vi "温度控制 - WK12.vi"(7 "CSM Name":string="WK1") -> ()   [LabVIEW 2017, in "UI-温度控制.lvlib"]
doc: "本范例执行串口读写操作。串口设置的参数必须匹配连接仪器或设备的参数。“VISA配置串口”VI可设置配置参数。前面板显示的控件可用于配置基本参数，如波特率、数据位和校验。VI会将VISA资源名称传递至其他VI以便执行相关操作。“VISA写入”函数将发送一个命令至串行设备，“VISA读取”函数将返回基于该命令的数据。“VISA关闭”函数可关闭该串行设备的引用。关闭引用十分重要，否则可能导致无法通过该端口进行进一步通信。"
uses:
  <userlib>/_NEVSTOP/Communicable State Machine(CSM)/Communicable State Machine.lvlib
  <userlib>/_NEVSTOP/Communicable State Machine(CSM)/addons/MassData-Parameter/CSM MassData Parameter Support.lvlib
  <userlib>/_NEVSTOP/Communicable State Machine(CSM)/addons/INI-Static-Variable-Support/INI-Static-Variable-Support.lvlib
  <userlib>/_NEVSTOP/Communicable State Machine(CSM)/addons/Watchdog/CSM Watchdog.lvlib
  <userlib>/_NEVSTOP/Communicable State Machine(CSM)/addons/Logger/CSM File Logger.lvlib
  e87f5527-76ec-45cd-8a15-2e3ba2958834.vi
  e40b3fcb-6c9f-41ae-97ff-bcb9991e0652.vi
  620e82e9-b677-4d25-b56c-4b090e123e3d.vi
  fecb341a-c865-4baa-9917-6b90415d6ef9.vi
  afd7753c-ea30-4e5b-9716-29bc73ab5d02.vi
  9a199716-2ffa-4f43-b9de-bb583d0dc84c.vi
  b5fe0464-1048-4df8-950b-6816aac68042.vi
  <userlib>/_NEVSTOP/Communicable State Machine(CSM)/_Polymophic/CSM - Replace Marks in Messages.vi
  7f493404-46e2-4a42-937c-85a599ffd008.vi
  3c0606d2-39f9-4349-a74d-1248628ec5a5.vi
  b1075206-a0bc-4c2c-8117-03daddfb89bc.vi
  12798cb0-d503-413b-8ceb-4a5576430bcb.vi
  22b4bb12-f94e-4276-9d0b-49463fdbebaf.vi
  87263e8e-d87a-4015-b0d9-f89f6746087b.vi
  45ac6a38-59b2-4408-864e-de2893445c95.vi
  3f8d9458-3e99-4457-8efa-55d1ef2330f2.vi
  bd3177e1-6bd6-42ad-a258-ed35146a2f34.vi
  acea6df9-f425-4d5c-b033-3243991d638c.vi
  611bdd8b-2aca-4a53-81a9-536b5b4081e0.vi
  6c66f1b3-0c4e-481a-bccf-761e4204c7a2.vi
  bd3fa8c0-2a07-4348-928a-5492c50b8d1d.vi
  bfd69444-e477-482d-b4ce-b6780147d2f5.vi
  3eee923a-0692-424c-8c25-dbf31775acba.vi
  026bd4a5-6a46-4a68-819b-9f168641a175.vi
  6fdd3ccc-b7af-4740-b642-363912b39baa.vi
  3bdb7142-561a-47bb-abd8-0318bec92597.vi
  dc7ef564-96da-43a3-866d-645d9c897f58.vi
  <vilib>/Instr/_visa.llb/VISA Configure Serial Port (Instr).vi
  6094d1ba-01c9-4f0f-81c2-2bfc5faa83cd.vi
  36fd150c-2ad9-4592-a276-8ca334c7aa56.vi
  f347ec19-a9ab-456c-bf02-8d1d7c992b68.vi
  6f01d93e-47d7-4c16-bfcb-79e48a01ebec.vi
  9b669b8c-733c-4058-8ee2-0fdaa3bce225.vi
  b7989555-3743-433e-92bc-1f24cc67f5f4.vi
  e0d25892-2f3c-4bdd-91b3-ce78b04bde2a.vi
  7ceba0d5-fd35-45f6-9e4f-db13be910fa9.vi
  e709ab76-91cd-483a-bfeb-5221a7f7e432.vi
  <userlib>/_NEVSTOP/Communicable State Machine(CSM)/addons/INI-Static-Variable-Support/_Support/instances/_CSM - Read File Logger Configuration - v1.0.vi
  <userlib>/_NEVSTOP/Communicable State Machine(CSM)/_Polymophic/CSM - Filter Duplicated Lines.vi
  <userlib>/_NEVSTOP/Communicable State Machine(CSM)/_Polymophic/Add State(s) to Queue By BOOL(Element).vi
  52a88361-96b9-4f42-83b5-2b3a91f6fe46.vi
  6e92e572-67e2-4f23-93e9-3f2621f8ebb2.vi
  fcc43e12-244c-4800-bcec-4b40395c6c4b.vi
  b77c82fb-bb1b-4fca-94e8-a2470f067fd9.vi
  cab45986-ae3d-44a0-b15a-916822da0a04.vi
  b63380f4-522f-43f9-8c86-ff87e18121f1.vi
  e181f527-371e-42fd-b1ab-20e25477ecf6.vi
  2a5f06fa-bc14-4be7-8a56-d3603e987429.vi
  Data ColndSave/Supports/Time and Data.ctl
  Data ColndSave/Data Collection and Save.lvlib
  Supports/Device Info.ctl
  a4ed0b2b-8fbd-453e-8bc8-e71f1ca0e4fa.vi
  967289fb-03de-4dd6-8fec-445893c11e8c.vi
panel:
  in  "停止":bool
  in  "温度显示":T1(tab)
  in  "温控开关 总":bool
  in  "跟随通道 1":T2
  in  "跟随通道 2":T2
  in  "通道":bool
  in  "温控温度 B":dbl=25.0 min=-10.0 max=50.0 step=0.1 format="%.2g"
  in  "温控温度 A":dbl=25.0 min=-10.0 max=50.0 step=0.1 format="%.2g"
  in  "温度":bool
  in  "跟随偏移 2":dbl min=-10.0 max=50.0 step=0.01 format="%#.2g"
  in  "是否跟随 2":bool
  in  "跟随偏移 1":dbl min=-10.0 max=50.0 step=0.01 format="%#.2g"
  in  "是否跟随 1":bool
  in  "打开串口":bool
  in  "温控串口":refnum<visa-resource-name>="COM18"
  out "TC2":waveform(dbl)[](graph)
  out "TC1":waveform(dbl)[](graph)
  in  "温控开关 2":bool
  in  "温控开关 1":bool
  in  "温控温度 2":dbl=25.0 min=-10.0 max=50.0 step=0.1 format="%.2g"
  out "实际温度 2":dbl=25.0 format="%.2g"
  out "实际温度 1":dbl=25.0 format="%.2g"
  in  "温控温度 1":dbl=25.0 min=-10.0 max=50.0 step=0.1 format="%.2g"
  in  "Fast Mode":bool
  in  "采集间隔":dbl=0.5 min=0.05 max=50.0 step=0.1 format="%.2g"
  out "Power 2":waveform(dbl)[](graph)
  out "Power 1":waveform(dbl)[](graph)
  out "输出状态 1":T3
  out "输出状态 2":T3
  in  "电源切换 2":bool
  in  "电源切换 1":bool
  in  "输出设置 2":T4={"输出模式"=enum."加热模式", "最大输出电压"=5.0} {"最大输出电压" min=0.0001 max=10.0}
  in  "输出设置 1":T4={"输出模式"=enum."加热模式", "最大输出电压"=5.0} {"最大输出电压" min=0.0001 max=10.0}
  in  "PID 1":T5={"PID类型"=enum."PID", "P"=0.05, "I"=20.0, "D"=2.0, "PID控制间隔"=100.0, "PID计算方法"=enum."最大正向输出"}
  in  "PID 2":T5={"PID类型"=enum."PID", "P"=0.05, "I"=20.0, "D"=2.0, "PID控制间隔"=100.0, "PID计算方法"=enum."最大正向输出"}
  in  "过压/过流 2":cluster{"过压保护阈值":dbl, "过流保护阈值":dbl}={"过压保护阈值"=6.0, "过流保护阈值"=3.0}
  in  "过压/过流 1":cluster{"过压保护阈值":dbl, "过流保护阈值":dbl}={"过压保护阈值"=6.0, "过流保护阈值"=3.0}
  in  "过温 2":T6={"过温保护开关"=TRUE, "过温保护低阈值"=5.0, "过温保护高阈值"=45.0, "最低设定温度"=5.0, "最高设定温度"=45.0, "温度限速"=45.0} {"温度限速" min=0.01}
  out "保护结果 2":T7={"过压保护结果"=enum."正常", "过流保护结果"=enum."正常", "过温保护结果"=enum."正常"}
  out "保护结果 1":T7={"过压保护结果"=enum."正常", "过流保护结果"=enum."正常", "过温保护结果"=enum."正常"}
  in  "过温 1":T6={"过温保护开关"=TRUE, "过温保护低阈值"=5.0, "过温保护高阈值"=45.0, "最低设定温度"=5.0, "最高设定温度"=45.0, "温度限速"=45.0} {"温度限速" min=1e-06; "最低设定温度" min=0.0001}
  in  "温控循环功能开启":bool
  in  "子程序？":bool
  out "温控-错误输出":errorcluster
  out "温控器设备型号":string
  out "State History":string
  # "温度快切"
  # "V"
  # "A"
  # "V"
  # "A"
  # "V"
  # "V"
  # "ms"
  # "ms"
  # "℃/s"
  # "℃/s"
  # "恢复，继续运行；\n如继续报错，请检查参数，可尝试关闭串口重新打开。"
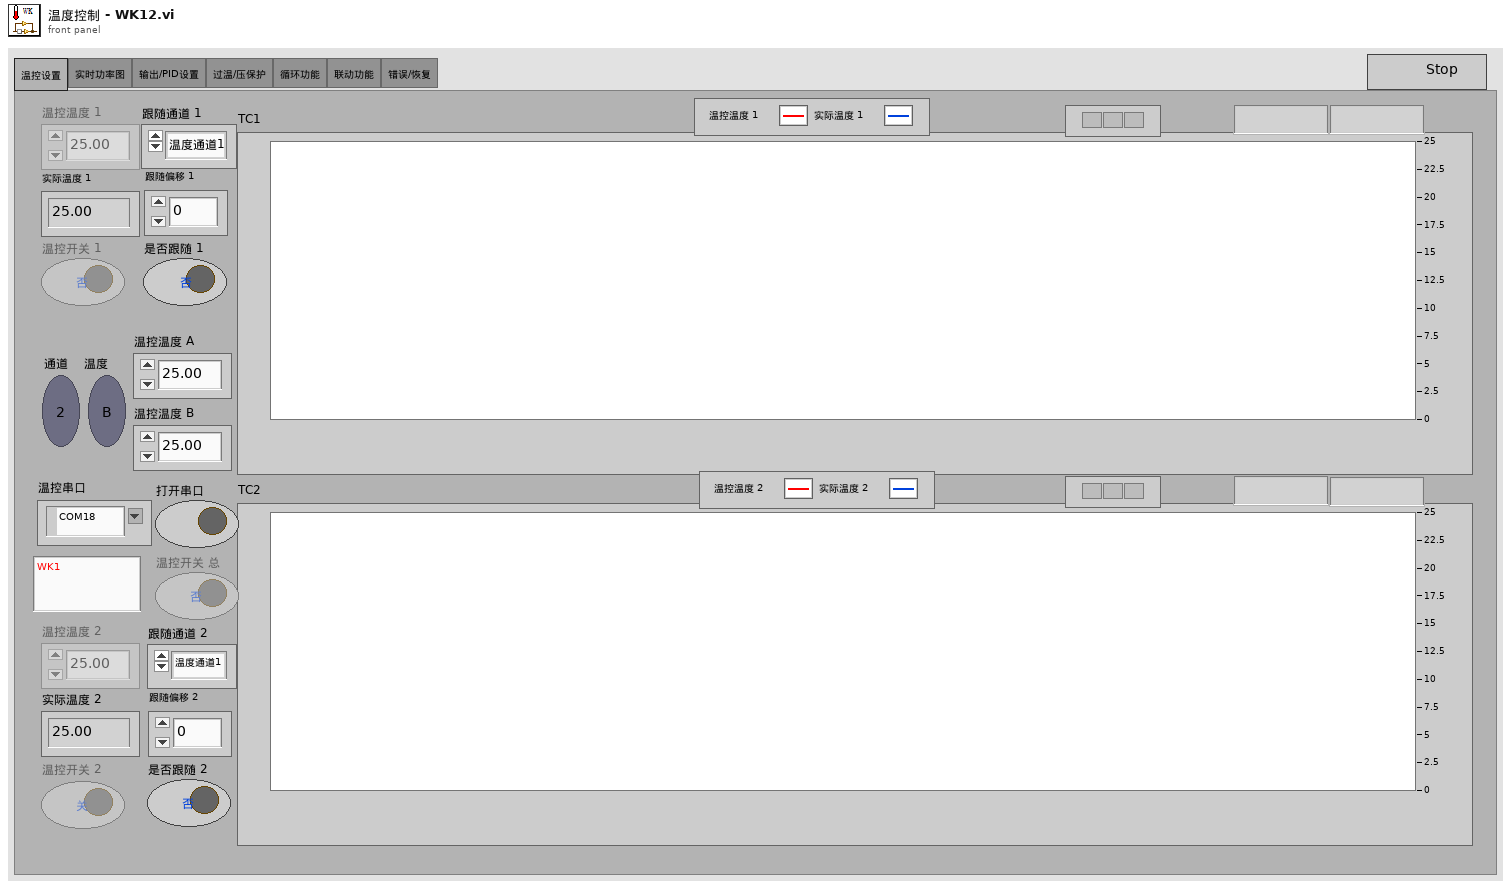
[diagram p1: front panel]
types:
  T1 = enum32{"温控设置", "实时功率图", "输出/PID设置", "过温/压保护", "循环功能", "联动功能", "错误/恢复"}
  T2 = typedef "UI-压力.lvlib/温度各项索引.ctl" = enum16{"温度通道1", "温度通道2", "温度通道3", "温度通道4", "温度通道5", "温度通道6", "温度通道7", "温度通道8", "TC1控制温度", "TC1实际温度", "TC1实际输出电压", "TC1实际输出电流", "TC1实际输出功率", "TC2控制温度", "TC2实际温度", "TC2实际输出电压", "TC2实际输出电流", "TC2实际输出功率", "压力(电压值)", "压力(g)", "步进电机位置", "温度", "湿度", "LD设定温度(度)", "LD实际温度(度)", "LD设定温度(脉冲值)", "LD实际温度(脉冲值)", "LD PWM(功率)"}
  T3 = cluster{"功率输出":enum16{"已关闭", "已打开"}, "实际输出电压":dbl, "实际输出电流":dbl}
  T4 = cluster{"输出模式":enum16{"致冷模式", "加热模式", "双向模式"}, "最大输出电压":dbl}
  T5 = cluster{"PID类型":enum16{"P", "PI", "PID"}, "P":dbl, "I":dbl, "D":dbl, "PID控制间隔":dbl, "PID计算方法":enum16{"位置式", "增量式", "最大正向输出", "最大负向输出"}}
  T6 = cluster{"过温保护开关":bool, "过温保护低阈值":dbl, "过温保护高阈值":dbl, "最低设定温度":dbl, "最高设定温度":dbl, "温度限速":dbl}
  T7 = cluster{"过压保护结果":enum16{"发现错误", "正常", "功能关闭"}, "过流保护结果":enum16{"发现错误", "正常", "功能关闭"}, "过温保护结果":enum16{"发现错误", "正常", "功能关闭"}}
  T8 = cluster{"Enable":bool, "Limit":cluster{"FileSize":i64, "FileNum":i32}, "Timestamp.Format":string, "AutoExit":bool}
  T9 = enum32{"Invalid", "Standard", "Closed", "Hidden", "Minimized", "Maximized"}
  T10 = enum32{"invalid app kind", "Development System", "Run Time System", "Student Edition", "Embedded LabVIEW", "Evaluation", "Custom"}
  T11 = typedef "Device Info.ctl" = cluster{"基本信息":cluster{"USB Port":refnum<visa-resource-name>, "采集间隔(s)":dbl}, "设备信息":cluster{"设备型号":string, "双通道设备？":bool}, "开关":cluster{"开关 1":bool, "开关 2":bool, "Fast Mode":bool}, "Control Temp":cluster{"Control Temp 1":dbl, "Control Temp 2":dbl}}
  T12 = cluster{"波特率":u32, "数据位":u16, "校验":enum16{"None", "Odd", "Even", "Mark", "Space"}, "停止位":u16, "流控制":u16}
  T13 = typedef "Communicable State Machine.lvlib/_CSM_Response Source Message.ctl" = cluster{"‘State":string, "’Arguments":string, "’Error":errorcluster}
  T14 = cluster{"Current VI Reference":refnum<vi>, "Close Panel on Exit?":bool}
  T15 = typedef "Data Collection and Save.lvlib/Time and Data.ctl" = cluster{"采集时间":timestamp, "Data":dbl[]}
  T16 = cluster{"Core":cluster{"Current VI Reference":refnum<vi>, "Close Panel on Exit?":bool}, "基本信息":cluster{"USB Port":refnum<visa-resource-name>, "采集间隔(s)":dbl}, "温控情况":cluster{"温控温度 1":dbl, "实际温度 1":dbl, "温控温度 2":dbl, "实际温度 2":dbl, "打开串口":bool}, "开关信息":cluster{"开关 1":bool, "开关 2":bool, "温控是否打开":bool}, "输出参数":cluster{"输出设置 1":cluster{"输出模式":enum16{"致冷模式", "加热模式", "双向模式"}, "最大输出电压":dbl}, "输出设置 2":cluster{"输出模式":enum16{"致冷模式", "加热模式", "双向模式"}, "最大输出电压":dbl}, "输出状态 1":cluster{"功率输出":enum16{"已关闭", "已打开"}, "实际输出电压":dbl, "实际输出电流":dbl, "实际输出功率":dbl}, "输出状态 2":cluster{"功率输出":enum16{"已关闭", "已打开"}, "实际输出电压":dbl, "实际输出电流":dbl, "实际输出功率":dbl}, "PID 1":cluster{"PID类型":enum16{"P", "PI", "PID"}, "P":dbl, "I":dbl, "D":dbl, "PID控制间隔":dbl, "PID计算方法":enum16{"位置式", "增量式", "最大正向输出", "最大负向输出"}}, "PID 2":cluster{"PID类型":enum16{"P", "PI", "PID"}, "P":dbl, "I":dbl, "D":dbl, "PID控制间隔":dbl, "PID计算方法":enum16{"位置式", "增量式", "最大正向输出", "最大负向输出"}}}, "保护":cluster{"过压/过流 1":cluster{"过压保护阈值":dbl, "过流保护阈值":dbl}, "过压/过流 2":cluster{"过压保护阈值":dbl, "过流保护阈值":dbl}, "保护结果 1":cluster{"过压保护结果":enum16{"发现错误", "正常", "功能关闭"}, "过流保护结果":enum16{"发现错误", "正常", "功能关闭"}, "过温保护结果":enum16{"发现错误", "正常", "功能关闭"}}, "保护结果 2":cluster{"过压保护结果":enum16{"发现错误", "正常", "功能关闭"}, "过流保护结果":enum16{"发现错误", "正常", "功能关闭"}, "过温保护结果":enum16{"发现错误", "正常", "功能关闭"}}, "过温 1":cluster{"过温保护开关":bool, "过温保护低阈值":dbl, "过温保护高阈值":dbl, "最低设定温度":dbl, "最高设定温度":dbl, "温度限速":dbl}, "过温 2":cluster{"过温保护开关":bool, "过温保护低阈值":dbl, "过温保护高阈值":dbl, "最低设定温度":dbl, "最高设定温度":dbl, "温度限速":dbl}}, "设备信息":cluster{"设备型号":string, "双通道设备？":bool}, "Time and Data":T15, "子程序":cluster{"子程序？":bool}}
  T17 = cluster{"过压/过流 1":cluster{"过压保护阈值":dbl, "过流保护阈值":dbl}, "过压/过流 2":cluster{"过压保护阈值":dbl, "过流保护阈值":dbl}, "保护结果 1":cluster{"过压保护结果":enum16{"发现错误", "正常", "功能关闭"}, "过流保护结果":enum16{"发现错误", "正常", "功能关闭"}, "过温保护结果":enum16{"发现错误", "正常", "功能关闭"}}, "保护结果 2":cluster{"过压保护结果":enum16{"发现错误", "正常", "功能关闭"}, "过流保护结果":enum16{"发现错误", "正常", "功能关闭"}, "过温保护结果":enum16{"发现错误", "正常", "功能关闭"}}, "过温 1":cluster{"过温保护开关":bool, "过温保护低阈值":dbl, "过温保护高阈值":dbl, "最低设定温度":dbl, "最高设定温度":dbl, "温度限速":dbl}, "过温 2":cluster{"过温保护开关":bool, "过温保护低阈值":dbl, "过温保护高阈值":dbl, "最低设定温度":dbl, "最高设定温度":dbl, "温度限速":dbl}}
  T18 = cluster{"输出设置 1":cluster{"输出模式":enum16{"致冷模式", "加热模式", "双向模式"}, "最大输出电压":dbl}, "输出设置 2":cluster{"输出模式":enum16{"致冷模式", "加热模式", "双向模式"}, "最大输出电压":dbl}, "输出状态 1":cluster{"功率输出":enum16{"已关闭", "已打开"}, "实际输出电压":dbl, "实际输出电流":dbl, "实际输出功率":dbl}, "输出状态 2":cluster{"功率输出":enum16{"已关闭", "已打开"}, "实际输出电压":dbl, "实际输出电流":dbl, "实际输出功率":dbl}, "PID 1":cluster{"PID类型":enum16{"P", "PI", "PID"}, "P":dbl, "I":dbl, "D":dbl, "PID控制间隔":dbl, "PID计算方法":enum16{"位置式", "增量式", "最大正向输出", "最大负向输出"}}, "PID 2":cluster{"PID类型":enum16{"P", "PI", "PID"}, "P":dbl, "I":dbl, "D":dbl, "PID控制间隔":dbl, "PID计算方法":enum16{"位置式", "增量式", "最大正向输出", "最大负向输出"}}}
  T19 = cluster{"温控温度 1":dbl, "实际温度 1":dbl, "温控温度 2":dbl, "实际温度 2":dbl, "打开串口":bool}
  T20 = cluster{"USB Port":refnum<visa-resource-name>, "采集间隔(s)":dbl}
  T21 = enum8{"Enabled", "Disabled", "Disabled and Grayed Out"}
  T22 = cluster{"控制温度":dbl, "时长(s)":dbl, "进度":dbl, "温控开关":bool}[]
  T23 = cluster{"PID类型":bool, "P":bool, "I":bool, "D":bool, "PID控制间隔":bool, "PID计算方法":bool}
  T24 = cluster{"过温保护开关":bool, "过温保护低阈值":bool, "过温保护高阈值":bool, "最低设定温度":bool, "最高设定温度":bool, "温度限速":bool}
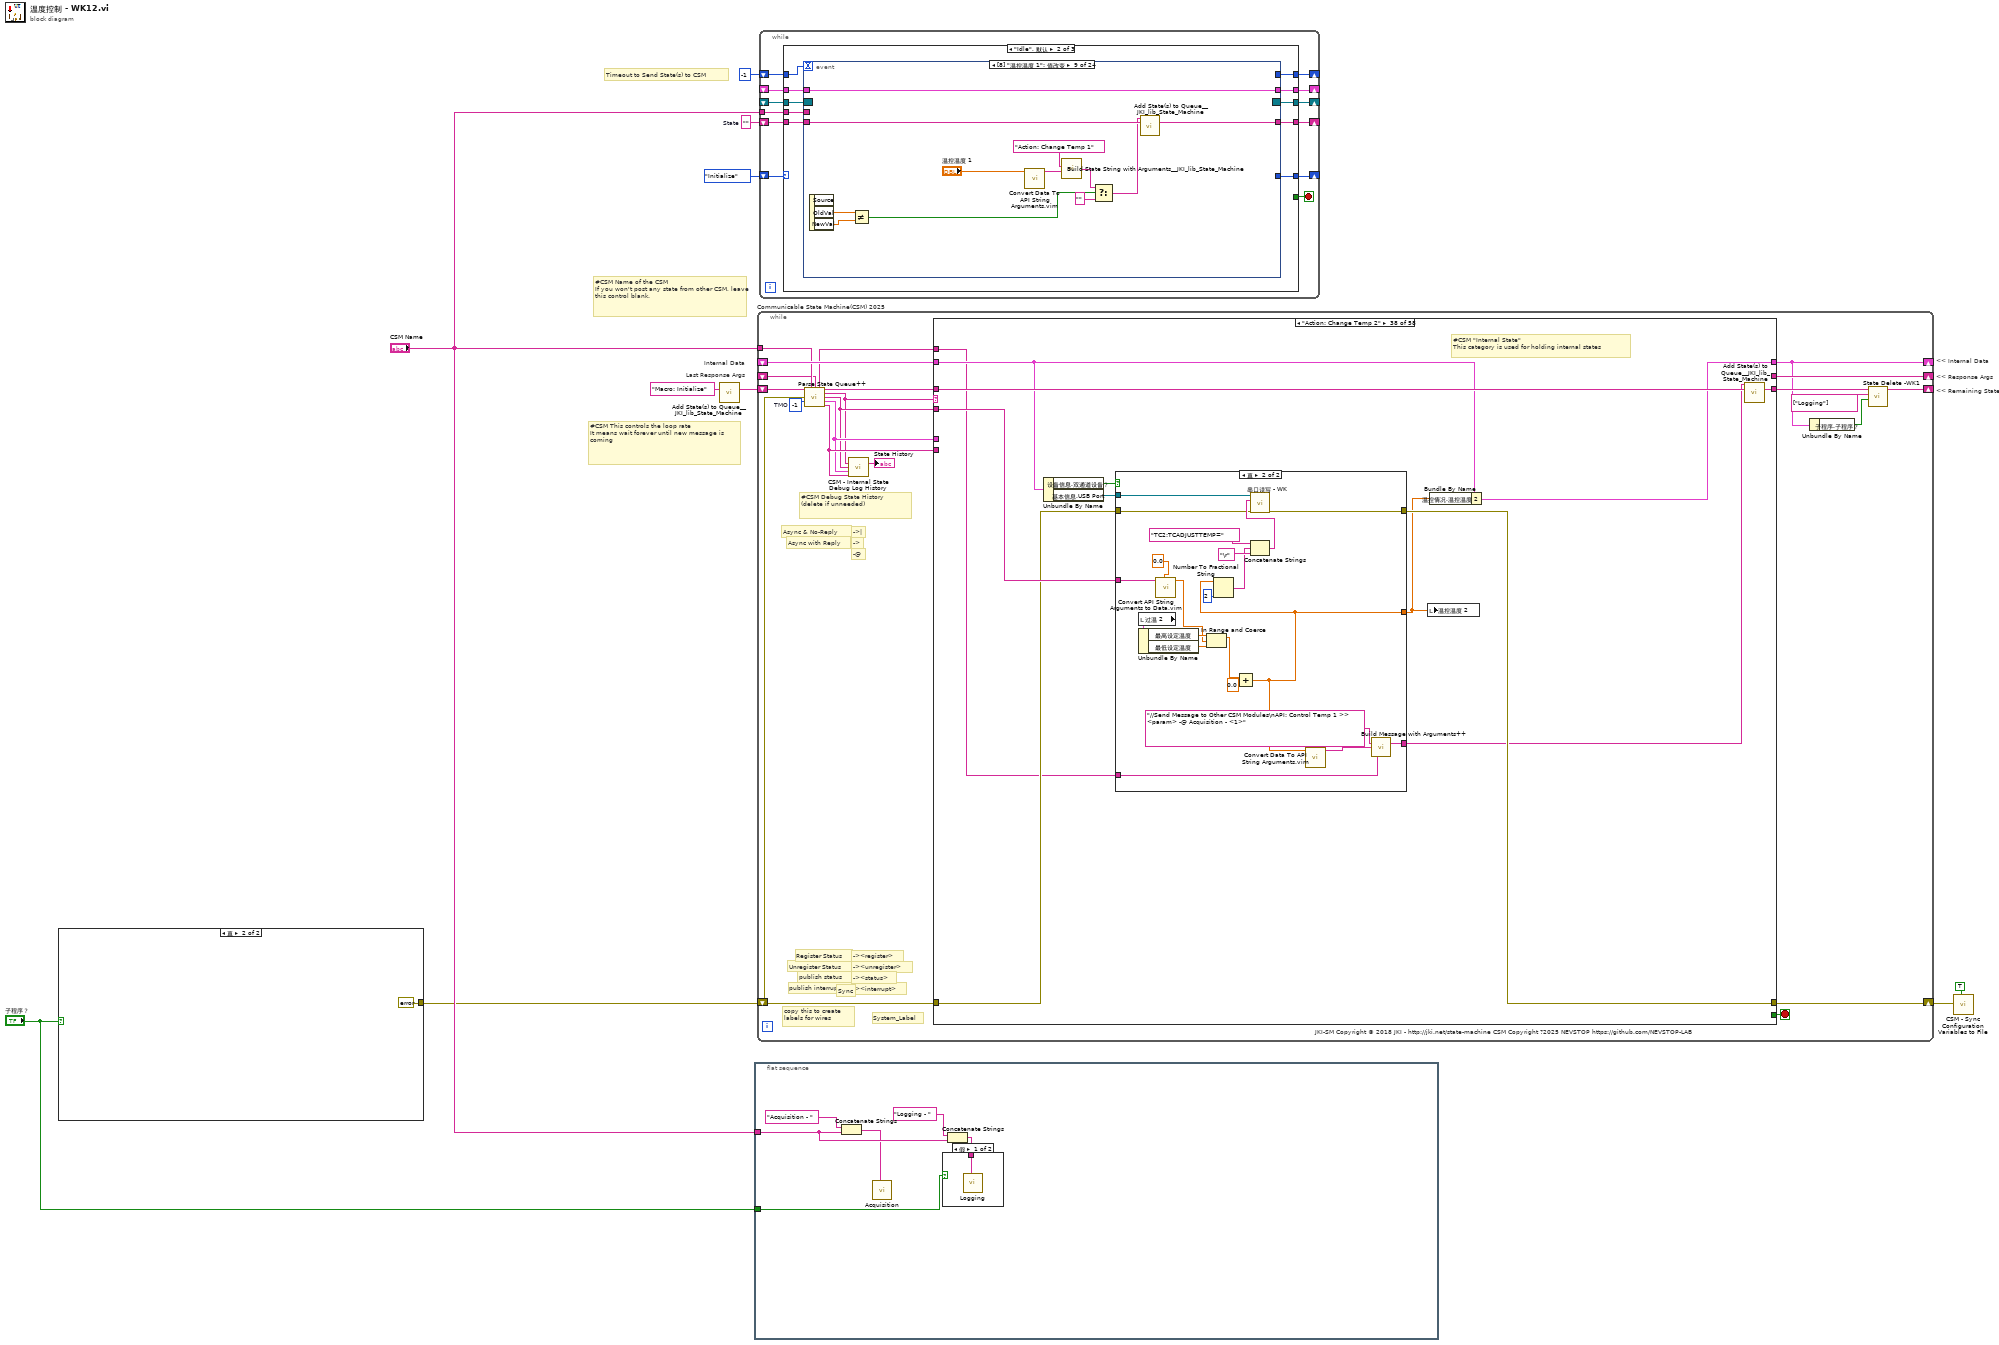
[diagram p0: block diagram]
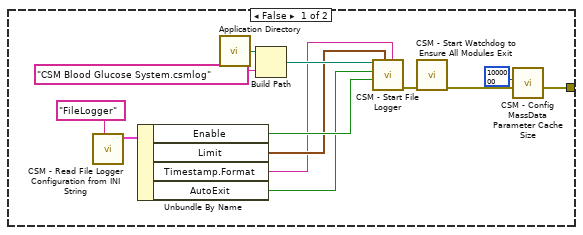
[diagram p2: hidden frame]
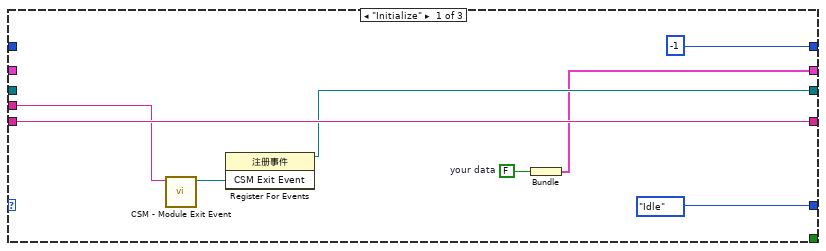
[diagram p4: hidden frame]
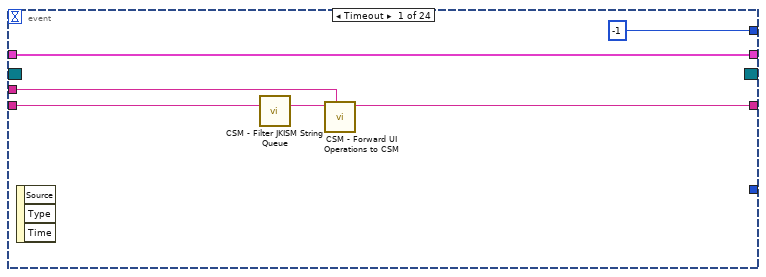
[diagram p5: hidden frame]
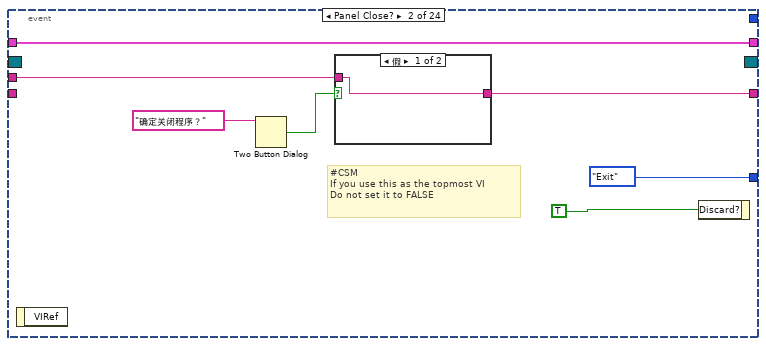
[diagram p6: hidden frame]
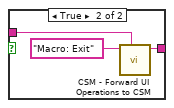
[diagram p7: hidden frame]
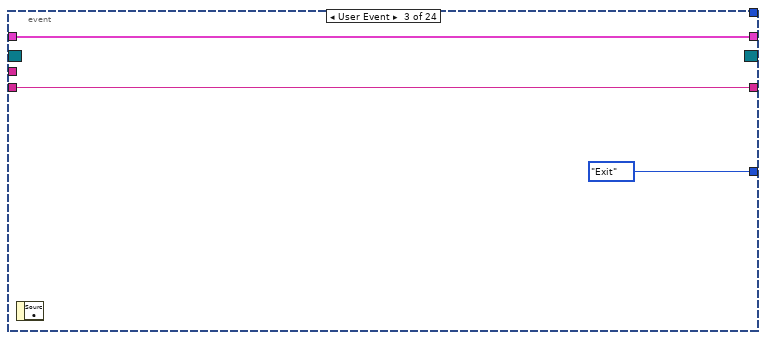
[diagram p8: hidden frame]
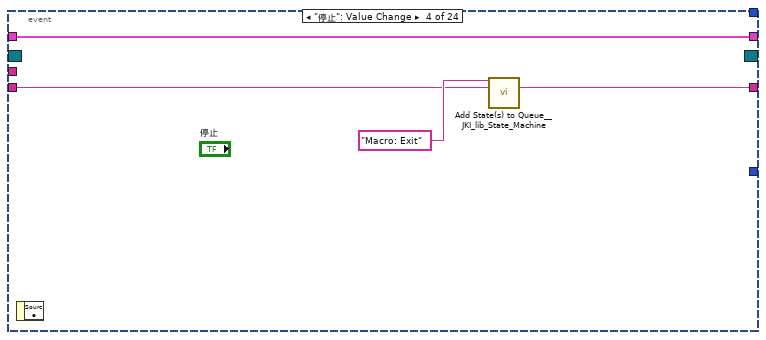
[diagram p9: hidden frame]
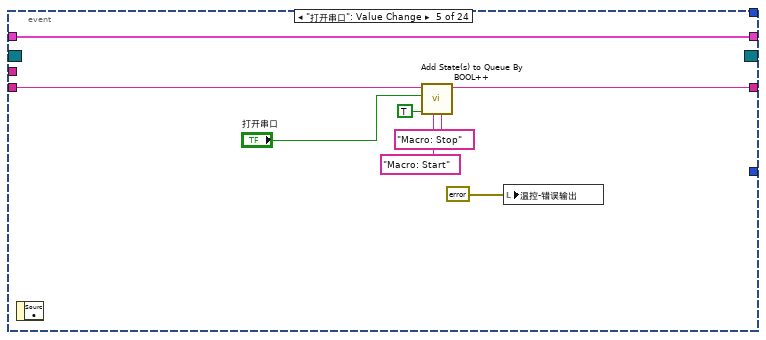
[diagram p10: hidden frame]
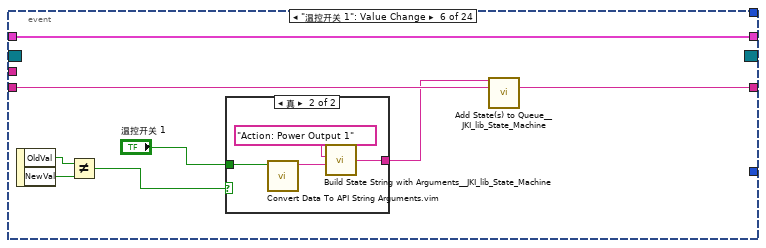
[diagram p11: hidden frame]
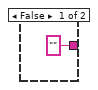
[diagram p12: hidden frame]
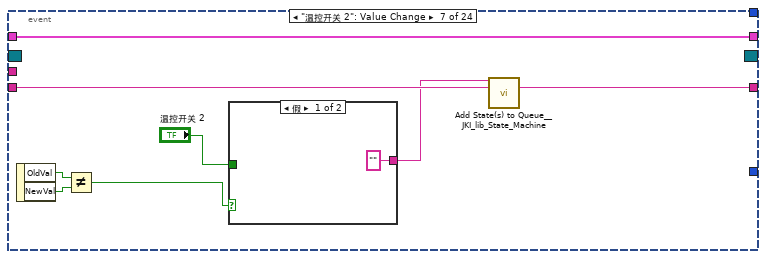
[diagram p13: hidden frame]
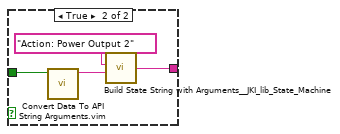
[diagram p14: hidden frame]
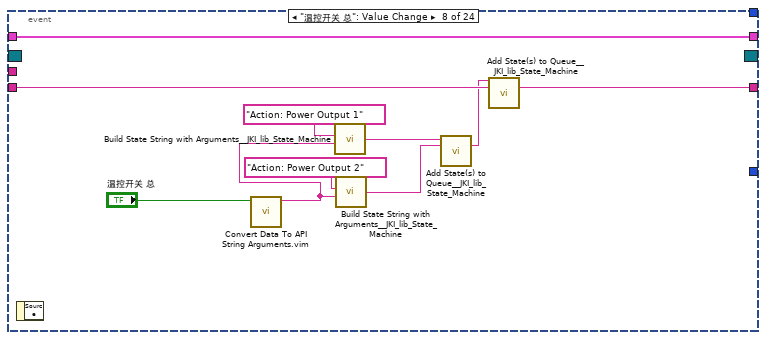
[diagram p15: hidden frame]
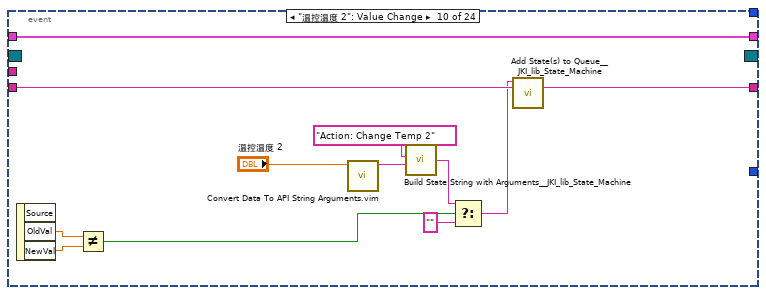
[diagram p16: hidden frame]
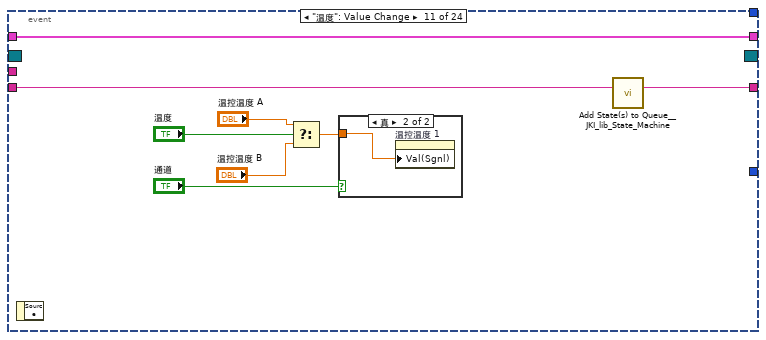
[diagram p17: hidden frame]
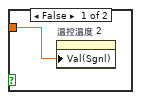
[diagram p18: hidden frame]
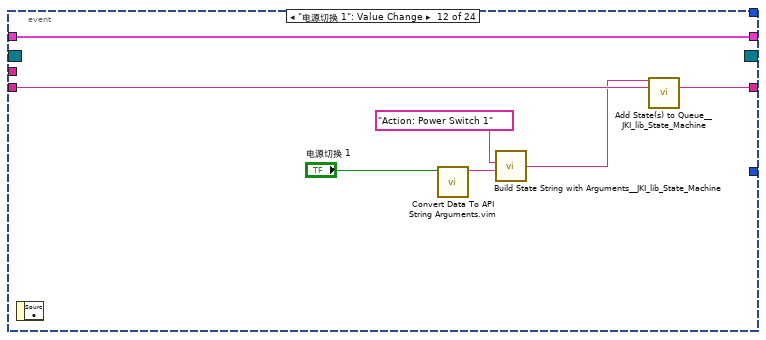
[diagram p19: hidden frame]
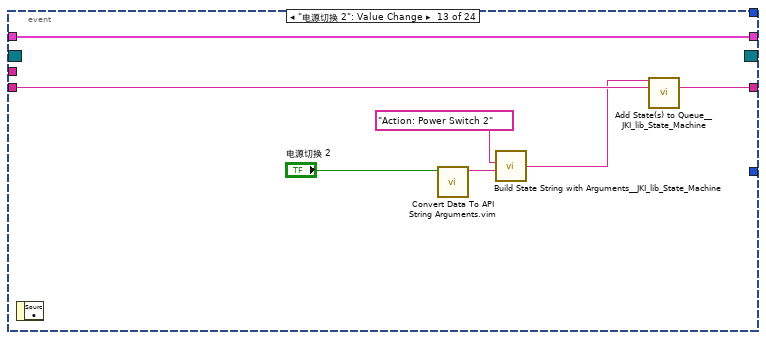
[diagram p20: hidden frame]
diagram:
  w9 = ""  # State
  # "Timeout to Send State(s) to CSM"
  # "Last Response Args"
  # "Internal Data"
  # "#CSM Name of the CSM\nIf you won't post any state from other CSM, leave this control blank."
  # "#CSM This controls the loop rate\nIt means wait forever until new message is coming"
  # "<< Internal Data"
  # "<< Response Args"
  # "<< Remaining States"
  n1 = case shown="真" "子程序？" {
    tunnel: [w21 errorcluster {"status"=FALSE, "code"=0, "source"=""} ("Error out")] -> w2
    frame False {
      n2 = call-poly <userlib>:"CSM - Read File Logger Configuration from INI String.vi"("Section Name(\"FileLogger\")"="FileLogger" ("Section Name(\"\" as Default)")) -> ("FileLogger Configuration-v1"=w15:T8)  [unwired: 7 in, 1 out]
      n3 = Unbundle By Name(w15) -> ("Enable"=w14:bool, "Limit"=w13:cluster{"FileSize":i64, "FileNum":i32}, "Timestamp.Format"=w11:string, "AutoExit"=w12:bool)
      n4 = call <vilib>:"Application Directory.vi"() -> ("Application Directory"=w20:path)
      n5 = Build Path(base path=w20, name or relative path="CSM Blood Glucose System.csmlog") -> (appended path=w18:path)
      n6 = call <userlib>:"CSM - Start File Logger.vi"("Timestamp Format"=w11, "Log Limit"=w13, "Watchdog? (T)"=w14, "Exit When All Module Exist? (F)"=w12, "Log File Path"=w18) -> ("error out"=w17:errorcluster)  [unwired: 4 in, 2 out]
      n7 = call <userlib>:"CSM - Start Watchdog to Ensure All Modules Exit.vi"("error in (no error)"=w17) -> ("error out"=w22:errorcluster)  [unwired: 10 in]
      n8 = call <userlib>:"CSM - Config MassData Parameter Cache Size.vi"("Error in"=w22, "Size (1M)"=1000000 ("size(1M)")) -> ("Error out"=w21:errorcluster)  [unwired: 9 in]
    }
    frame True {
    }
  }
  n9 = call <vilib>:"Add State(s) to Queue__JKI_lib_State_Machine.vi"("State(s) in (\"\")"="Macro: Initialize" ("Init State(\"Macro: Initialize\")")) -> ("States Out"=w6:string)  [unwired: 14 in]
  n10 = flat-sequence {
    tunnel: "CSM Name" -> [w27]
    tunnel: "子程序？" -> [w25]
    frame #0 {
      n11 = Concatenate Strings("Acquisition - " ("Name(\"\" to use uuid)"), w27) -> (w26:string)
      n12 = call "Acquisition.vi"("Name (\"\" to Use UUID)"=w26) -> ()  [unwired: 11 in]
      n13 = Concatenate Strings("Logging - " ("Name(\"\" to use uuid)"), w27) -> (w28:string)
      n14 = case shown="假" w25 {
        tunnel: w28 -> [w31 _]
        frame False {
          n15 = call "Logging.vi"("CSM Name"=w31) -> ()  [unwired: 11 in]
        }
        frame True {
        }
      }
    }
  }
  n16 = while "Communicable State Machine(CSM) 2025" {
    shift-right: [w33] -> _
    shift-left: _ -> [w48]
    shift-right: [w50] -> w4
    shift-left: w2 -> [w39]
    shift-right: [w35] -> _
    shift-left: w6 -> [w51]
    tunnel: "CSM Name" -> [w45]
    shift-right: [w46] -> _
    shift-left: _ -> [w40]
    stop <- w49 stop-if-true
    w47 = -1  # TMO
    # "#CSM Debug State History\n(delete if unneeded)"
    # "-><interrupt>"
    # "-><status>"
    # "-><unregister>"
    # "-><register>"
    # "-@"
    # "->"
    # "->|"
    # "publish interrupt"
    # "publish status"
    # "Unregister Status"
    # "Register Status"
    # "Sync"
    # "Async with Reply"
    # "Async & No-Reply"
    # "JKI-SM Copyright © 2018 JKI - http://jki.net/state-machine CSM Copyright ?2025 NEVSTOP https://github.com/NEVSTOP-LAB"
    # "copy this to create labels for wires"
    # "System_Label"
    n17 = call <userlib>:"Parse State Queue++.vi"("State Queue"=w51, "Name (\"\" to Use UUID)"=w45, "Response Arguments"=w40, "Previous Error"=w39, "Dequeue (1 ms)"=w47) -> ("Name Used"=w37:string, "Remaining States"=w52:string, "Current State"=w41:string, "Arguments"=w42:string, "Additional Information"=w43:T13, "Source CSM"=w44:string)  [unwired: 5 in]
    n18 = call <userlib>:"CSM - Internal State Debug Log History.vi"("State"=w41, "Arguments (\"\")"=w42, ">> Response Source Message >>"=w43, "Source (\"\")"=w44) -> ("Debug Log"=→"State History":string)  [unwired: 11 in]
    n19 = case shown="\"Action: Change Temp 2\"" w41 {
      selector: w41 -> [_ _ _ w64 _ _ _ _ _ _ _ _ _ _ _ _ _ _ _ _ _ _ _ _ _ _ _ _ _ _ _ _ _ _ _ _ _ _ _ _ _ _ _ _ _ _ _ _ _ _ _ _ _ _ _ _ _ _]
      tunnel: w52 -> [w53 w57 w60 w68 w73 w79 w104 w110 w116 w126 w133 w145 w149 w152 w170 w210 w227 w229 w250 w252 w284 w310 w341 w372 w429 w503 w533 w537 w543 w588 w601 w630 w642 w645 w663 w681 w706 w718 w757 w772 w781 w808 w838 w883 w928 w974 w1020 w1049 w1068 w1070 w1078 w1086 w1099 w1106 w1119 w1132 w1144 w1149]
      tunnel: w42 -> [_ _ _ _ _ w78 w100 w107 w113 w120 _ _ _ _ _ w203 _ _ _ _ _ _ _ _ _ _ _ _ _ _ _ _ _ _ w655 w673 w685 w712 w750 w765 w780 w807 w837 w882 w927 w973 w1019 w1048 _ w1073 w1081 w1089 w1096 _ _ w1130 _ _]
      tunnel: w48 -> [w55 w56 w58 w66 w72 w84 w102 w108 w114 w124 w132 w139 w147 w150 _ w194 w222 w230 w245 w256 w275 w303 w315 w346 w406 w484 w507 w535 w541 w567 w597 w634 w637 w643 w652 w670 w698 w715 w747 w762 w776 w803 w831 w874 w920 w967 w1011 w1040 w1067 w1075 w1083 w1091 w1097 w1104 w1111 w1134 w1142 w1148]
      tunnel: [_ _ _ w61 w74 errorcluster {"status"=FALSE, "code"=0, "source"=""} ("error out") w97 w105 w111 w127 _ _ _ _ _ _ w223 w231 w251 w257 w263 w287 w312 w343 w375 w450 w534 _ _ w549 w598 w635 _ _ w650 w668 w696 w713 w745 w760 w773 w800 w832 w877 w922 w968 w1014 w1043 _ w1076 w1084 w1092 w1103 _ _ w1135 _ w1150] -> w50
      tunnel: w39 -> [_ _ _ w62 w74 w82 w98 w106 w112 _ _ _ _ _ _ _ w224 w231 w251 w257 w273 w288 w313 w344 w376 w451 w534 _ _ w549 w599 w635 _ _ w656 w674 w694 w711 w751 w766 w774 w801 w833 w878 w923 w969 w1015 w1044 _ w1076 w1084 w1092 w1103 _ _ w1135 _ w1150]
      tunnel: [w54 w57 w59 w67 w73 w80 w103 w109 w115 w125 w133 w144 w148 w151 w169 w211 w226 w228 w249 w253 w285 w311 w342 w373 w430 w504 w532 w536 w542 w587 w600 w631 w641 w644 w662 w680 w705 w717 w756 w771 w782 w809 w839 w884 w929 w975 w1021 w1050 w1068 w1071 w1079 w1087 w1100 w1105 w1118 w1133 w1143 w1149] -> w36
      tunnel: [_ _ _ _ _ _ TRUE _ _ _ _ _ TRUE _ _ _ _ _ _ _ _ _ _ _ _ _ _ _ _ _ _ _ _ _ _ _ _ _ _ _ _ _ _ _ _ _ _ _ _ _ _ _ _ _ _ _ _ _] -> w49
      tunnel: [w55 w56 w58 w66 w72 w84 w102 w108 w114 w123 w132 w143 w147 w150 w168 w195 w222 w230 w245 w256 w261 w302 w314 w371 w404 w483 w507 w535 w541 w561 w596 w634 w637 w643 w651 w669 w697 w714 w746 w761 w775 w802 w827 w873 w918 w963 w1012 w1041 w1067 w1075 w1083 w1091 w1093 w1104 w1111 w1134 w1142 w1148] -> w33
      tunnel: w44 -> [_ _ _ _ _ w77 _ _ _ w121 _ _ _ _ _ _ _ _ _ _ _ _ _ _ _ _ _ _ _ _ _ _ _ _ _ _ _ _ _ _ _ _ _ _ _ _ _ _ _ _ _ _ _ _ _ _ _ _]
      tunnel: w43 -> [_ _ _ _ _ w76 _ _ _ w122 _ _ _ _ _ _ _ _ _ _ _ _ _ _ _ _ _ _ _ _ _ _ _ _ _ _ _ _ _ _ _ _ _ _ _ _ _ _ _ _ _ _ _ _ _ _ _ _]
      tunnel: [_ _ _ "" w69 _ _ _ _ _ _ _ _ _ _ _ _ _ _ _ _ _ _ _ _ _ _ _ _ _ _ _ _ _ _ _ _ _ _ _ _ _ _ _ _ _ _ _ _ _ _ _ _ _ _ _ _ _] -> w46
      tunnel: w37 -> [_ _ _ w63 _ _ w99 _ _ _ _ _ _ _ w160 _ w220 _ _ _ _ _ _ _ _ _ _ _ w539 w562 _ w632 w640 _ _ _ w682 w707 _ _ _ _ _ _ _ _ _ _ _ w1072 w1080 w1088 w1101 _ w1107 w1128 w1141 _]
      frame "", "Idle" {
        # "#CSM \"Idle/Event Handler\"\nexecutes when the state queue is empty"
        n20 = call <vilib>:"Add State(s) to Queue__JKI_lib_State_Machine.vi"("State(s) in (\"\")"=w53) -> ("States Out"=w54:string)  [unwired: 14 in]
      }
      frame "CSM Documentation" {
        # "#CSM State Syntax\n\n// Comment line, all text to the right of “//” will be ignored\n// Local Message Example\nDoSth: DoA >> Arguments\n\n// Sync Call Example\nAPI: xxxx >> Arguments -@ TargetModule\n\n// Async Call Example\nAPI: xxxx >> Arguments -> TargetModule\n\n// Async Call without Reply Example\nAPI: xxxx >> Arguments ->| TargetModule\n\n// Broadcast normal status:\nStatus >> StatusArguments  -><status>\n\n// Broadcast Interrupt status:\nInterrupt >> StatusArguments  -><interrupt>\n\n// Register Source Module's status to Handler Module\nStatus@Source Module >> Handler Module@Handler Module -><register>\n\n// Unegister Source Module's status\nStatus@Source Module >> Handler Module -><unregister>"
        # "#CSM README FIRST\n\nCommunicable State Machine(CSM) is a LabVIEW application framework that builds upon JKI State Machine(JKISM). It follows the pattern of JKISM and extends the keywords to describe message communication between modules, including concepts such as Sync-Message, Async-Message, Subscription/Unsubscription of status - essential elements for creating reusable code modules. For more information, please visit the CSM wiki: https://nevstop-lab.github.io/CSM-Wiki/\n\nFor instructions on JKI State Machine, visit: \n    http://jki.net/state-machine/\nFor information about CSM, visit: \n    https://github.com/NEVSTOP-LAB"
        # "#CSM \"Documentation\"\nCase for holding CSM Documenation"
      }
      frame "---------- Core ----------" {
        # "#CSM \"Category Seperator\"\nDo not put any code in this frame."
        n21 = call <vilib>:"Add State(s) to Queue__JKI_lib_State_Machine.vi"("State(s) in (\"\")"=w60) -> ("States Out"=w59:string)  [unwired: 14 in]
      }
      frame Default {
        # "#CSM \"Default\"\nthis is used to capture unhandled states and typos"
        n22 = call <userlib>:"CSM Unhandled State Error.vi"("error in (no error)"=w62, "Undefined State"=w64, "CSM Name"=w63) -> ("error out"=w61:errorcluster)  [unwired: 8 in]
        n23 = call <vilib>:"Add State(s) to Queue__JKI_lib_State_Machine.vi"("State(s) in (\"\")"=w68) -> ("States Out"=w67:string)  [unwired: 14 in]
      }
      frame "VI Reference" {
        n24 = Unbundle By Name(w72) -> ("Core"=w71:T14)
        n25 = Unbundle By Name(w71) -> ("Current VI Reference"=w70:refnum<vi>)
        n26 = call <userlib>:"CSM - Convert Data to HexStr.vi"("Variant"=w70) -> ("HEX String (0-9,A-F)"=w69:string)  [unwired: 8 in]
      }
      frame "Error Handler" {
        # "#CSM \"Error Handler\"\nYou can also output any states to clean-up after errors occur"
        # "Clear error"
        n27 = case shown="无错误" w82 {
          selector: w82 -> [_ w91]
          tunnel: [w89 w93] -> w81
          tunnel: w79 -> [w89 w92]
          tunnel: w78 -> [w88 _]
          tunnel: w77 -> [_ _]
          tunnel: w76 -> [_ _]
          tunnel: [w86 w91] -> w75
          frame No Error {
            n28 = call <userlib>:"CSM - Convert Argument to Error.vi"("Argument"=w88) -> ("Error"=w87:errorcluster)  [unwired: 4 in]
            n29 = flat-sequence {
              tunnel: w87 -> [w90]
              tunnel: [w90] -> w86
              frame #0 {
                # "#CSM External Error Handler Case\nUsually, it's because This CSM register others' \"Error Occurred\" status with \"Error Handler\". If other CSM have any error, the error will be passed here for central handling."
              }
            }
          }
          frame Error {
            # "#CSM Internal Error Handler Case \nIf any error Occurred, \"Error Occurred\" \nstatus update will be broadcasted to system.\nParameter is Error Cluster."
            n30 = call <userlib>:"CSM - Convert Error to Argument.vi"("Error"=w91) -> ("Argument"=w95:string)  [unwired: 4 in]
            n31 = call <vilib>:"Build State String with Arguments__JKI_lib_State_Machine.vi"("Arguments (\"\")"=w95, "State"="Error Occurred" ("Status with Arguments")) -> ("State with Arguments"=w94:string)  [unwired: 4 in]
            n32 = call <userlib>:"CSM - Broadcast Status Change.vi"("Status With Arguments"=w94, "State Queue"=w92) -> ("Remaining States"=w93:string)  [unwired: 13 in]
          }
        }
        "温控-错误输出" <- w75
        n33 = call <vilib>:"Add State(s) to Queue__JKI_lib_State_Machine.vi"("State(s) in Front (\"\")"="// Post Error States", "State(s) in (\"\")"=w81) -> ("States Out"=w80:string)  [unwired: 13 in]
      }
      frame "Critical Error" {
        # "#CSM \"Critical Error\"\nWhen any un-recoverable error occurs, CSM goes into this case."
        # "#CSM Stop in Critical Error\nWhen Critical Error occurs, Stop the loop immediately. Do NOT change this unless you fully understand the impact."
        n34 = call <userlib>:"CSM Critical Error.vi"("error in (no error)"=w98, "Arugments (As Reason)"=w100, "CSM Name"=w99) -> ("error out"=w97:errorcluster)  [unwired: 8 in]
        n35 = call <vilib>:"Add State(s) to Queue__JKI_lib_State_Machine.vi"("State(s) in (\"\")"=w104) -> ("States Out"=w103:string)  [unwired: 14 in]
      }
      frame "Target Timeout Error" {
        # "#CSM \"Target Timeout Error\"\nWhen This CSM could not get the sync-call response in time, This CSM goes into this case."
        n36 = call <userlib>:"CSM Target Timeout Error.vi"("error in (no error)"=w106, "Arguments (As CSM Name)"=w107) -> ("error out"=w105:errorcluster)  [unwired: 9 in]
        n37 = call <vilib>:"Add State(s) to Queue__JKI_lib_State_Machine.vi"("State(s) in (\"\")"=w110) -> ("States Out"=w109:string)  [unwired: 14 in]
      }
      frame "Target Error" {
        # "#CSM \"Target Error\"\nWhen This CSM try to communicate with an un-existed CSM, This CSM goes into this case."
        n38 = call <userlib>:"CSM Target Error.vi"("error in (no error)"=w112, "Arguments (As CSM Name)"=w113) -> ("error out"=w111:errorcluster)  [unwired: 9 in]
        n39 = call <vilib>:"Add State(s) to Queue__JKI_lib_State_Machine.vi"("State(s) in (\"\")"=w116) -> ("States Out"=w115:string)  [unwired: 14 in]
      }
      frame "Async Response", "Response" {
        n40 = Unbundle(w122) -> ("‘State"=w119:string, "’Arguments"=w118:string, "’Error"=w117:errorcluster)
        n41 = case shown="默认" w119 {
          tunnel: [w128] -> w125
          tunnel: w126 -> [w129]
          tunnel: [w131] -> w123
          tunnel: w124 -> [w131]
          tunnel: [w130] -> w127
          tunnel: w117 -> [w130]
          tunnel: w121 -> [_]
          tunnel: w120 -> [_]
          tunnel: w118 -> [_]
          frame 默认 {
            # "#CSM \"Async Response\"\nHandle Async-call Response (\"Async Response\" for ->)"
            # "#CSM \"Response\"\nHandle Sync-call Response (\"Response\" for -@)"
            # "#CSM Response Comments\nAfter Message is executed, CSM goes to this state for receive the response.\n    For Async Message(->), \"Async Response\" is used. This CSM will goes to \"Async Message Posted\" immediately and receive the \"Async Response\" after the callee finishes the message.\n    For Sync Message(@),  This CSM will wait until the message is done and immediately goes to \"Response\""
            n42 = call <vilib>:"Add State(s) to Queue__JKI_lib_State_Machine.vi"("State(s) in (\"\")"=w129) -> ("States Out"=w128:string)  [unwired: 14 in]
          }
        }
      }
      frame "Async Message Posted" {
        # "#CSM \"Async Message Posted\"\nAfter Async Message is posted (-> or ->| ), CSM goes to this state for post-action.\nYou can use Argument - State to tell which Async Message is called."
      }
      frame "Initialize Core Data" {
        # "#CSM \"Initialize Core Data\"\nThis is used to determine panel behavior on exit"
        # "originally closed?"
        # "exe?"
        # "If panel starts closed or is an EXE, then close it when we exit"
        n43 = property class="VI"() -> ("FP.State"=w136:T9)  [unwired: 2 in, 2 out]
        n44 = property class="App"() -> ("App.Kind"=w142:T10)  [unwired: 2 in, 2 out]
        n45 = control-ref of="Current VI Reference"() -> (w137:refnum<vi>)
        n46 = Equal?(x=w136, y=T9."Closed" ("Front Panel Window:State")) -> (x = y?=w134:bool)
        n47 = Equal?(x=w142, y=T10."Run Time System" ("Application:Kind")) -> (x = y?=w140:bool)
        n48 = Or(x=w134, y=w140) -> (x .or. y?=w138:bool)
        n49 = Bundle By Name(cluster=w139, "Core.Current VI Reference"=w137, "Core.Close Panel on Exit?"=w138) -> (w143:T16)
        n50 = call <vilib>:"Add State(s) to Queue__JKI_lib_State_Machine.vi"("State(s) in (\"\")"=w145) -> ("States Out"=w144:string)  [unwired: 14 in]
      }
      frame "Exit" {
        # "#CSM \"Exit\"\nCase for exiting the loop. No errors that occur here will be handled."
        n51 = call <vilib>:"Add State(s) to Queue__JKI_lib_State_Machine.vi"("State(s) in (\"\")"=w149) -> ("States Out"=w148:string)  [unwired: 14 in]
      }
      frame "---------- Data ----------" {
        # "#CSM \"Category Seperator\"\nDo not put any code in this frame."
        n52 = call <vilib>:"Add State(s) to Queue__JKI_lib_State_Machine.vi"("State(s) in (\"\")"=w152) -> ("States Out"=w151:string)  [unwired: 14 in]
      }
      frame "Data: Initialize" {
        w155 = cluster{"子程序？":bool} {"子程序？"=FALSE}  # 子程序
        w161 = cluster{"开关 1":bool, "开关 2":bool, "温控是否打开":bool} {"开关 1"=FALSE, "开关 2"=FALSE, "温控是否打开"=FALSE}  # 开关信息
        w162 = T15 {"采集时间"=timestamp(0 s since 1904-01-01), "Data"=[]}  # Time and Data
        w164 = T17 {"过压/过流 1"={"过压保护阈值"=6.0, "过流保护阈值"=3.0}, "过压/过流 2"={"过压保护阈值"=6.0, "过流保护阈值"=3.0}, "保护结果 1"={"过压保护结果"=enum."正常", "过流保护结果"=enum."正常", "过温保护结果"=enum."正常"}, "保护结果 2"={"过压保护结果"=enum."正常", "过流保护结果"=enum."正常", "过温保护结果"=enum."正常"}, "过温 1"={"过温保护开关"=FALSE, "过温保护低阈值"=5.0, "过温保护高阈值"=45.0, "最低设定温度"=5.0, "最高设定温度"=45.0, "温度限速"=0.0}, "过温 2"={"过温保护开关"=FALSE, "过温保护低阈值"=5.0, "过温保护高阈值"=45.0, "最低设定温度"=5.0, "最高设定温度"=45.0, "温度限速"=0.0}}  # 保护
        w163 = cluster{"设备型号":string, "双通道设备？":bool} {"设备型号"="", "双通道设备？"=FALSE}  # 设备信息
        w165 = T18 {"输出设置 1"={"输出模式"=enum."加热模式", "最大输出电压"=5.0}, "输出设置 2"={"输出模式"=enum."加热模式", "最大输出电压"=5.0}, "输出状态 1"={"功率输出"=enum."已关闭", "实际输出电压"=0.0, "实际输出电流"=0.0, "实际输出功率"=0.0}, "输出状态 2"={"功率输出"=enum."已关闭", "实际输出电压"=0.0, "实际输出电流"=0.0, "实际输出功率"=0.0}, "PID 1"={"PID类型"=enum."PID", "P"=0.05, "I"=20.0, "D"=2.0, "PID控制间隔"=0.1, "PID计算方法"=enum."最大正向输出"}, "PID 2"={"PID类型"=enum."PID", "P"=0.05, "I"=20.0, "D"=2.0, "PID控制间隔"=0.1, "PID计算方法"=enum."最大正向输出"}}  # 输出参数
        w166 = T19 {"温控温度 1"=25.0, "实际温度 1"=25.0, "温控温度 2"=25.0, "实际温度 2"=25.0, "打开串口"=FALSE}  # 温控情况
        w157 = T20 {"USB Port"="COM1", "采集间隔(s)"=0.5}  # 基本信息
        w167 = T14 {"Current VI Reference"=refnum, "Close Panel on Exit?"=FALSE}  # Core
        # "#CSM \"Data: Initialize\"\nInitialize the shift-register data, here.\n(data names are defined by what you wire into the bundle function)"
        # "#CSM do not delete - used by framework"
        # "#CSM Expand Bundle to add new data elements to shift register data."
        # "#CSM Data names and types of shift register data are defined by this bundle."
        n53 = call "CSM - Read Cluster Elements From Session.vim"("Section Name (\"\" as Default)"=w160, "Cluster"=w157) -> ("Cluster out"=w158:T20)  [unwired: 6 in, 1 out]
        n54 = local read "子程序？"() -> (w154:bool)
        n55 = Select(t=w158, s=TRUE, f=w157) -> (s? t:f=w156:T20)
        n56 = Bundle By Name(cluster=w155, "子程序？"=w154) -> (w153:cluster{"子程序？":bool})
        n57 = Bundle("Core"=w167, "基本信息"=w156, "温控情况"=w166, "开关信息"=w161, "输出参数"=w165, "保护"=w164, "设备信息"=w163, "Time and Data"=w162, "子程序"=w153) -> (w168:T16)  [unwired: 1 in]
        n58 = call <vilib>:"Add State(s) to Queue__JKI_lib_State_Machine.vi"("State(s) in (\"\")"=w170) -> ("States Out"=w169:string)  [unwired: 14 in]
      }
      frame "Data: Update Indicators" {
        w191 = dbl[] [] ("数组")
        w209 = T15 {"采集时间"=timestamp(0 s since 1904-01-01), "Data"=[]}  # Time and Data
        n59 = Unbundle By Name(w194) -> ("输出参数.输出状态 1.功率输出"=w193:enum16{"已关闭", "已打开"}, "输出参数.输出状态 2.功率输出"=w192:enum16{"已关闭", "已打开"}, "设备信息.双通道设备？"=w188:bool)
        n60 = call "CSM - Convert Argument to MassData.vim"("Type"=w209, "MassData Argument"=w203) -> ("Data"=w196:T15)  [unwired: 6 in, 1 out]
        n61 = Index Array(array=w191, index="跟随通道 1") -> (element=w207:dbl)
        n62 = Index Array(array=w191, index="跟随通道 2") -> (element=w206:dbl)
        n63 = Compound Arithmetic op=AND ("复合运算")("是否跟随 2", w188) -> (w190:bool)
        n64 = Unbundle By Name(w196) -> ("Data"=w197:dbl[])
        n65 = case shown="真" "是否跟随 1" {
          tunnel: w207 -> [_ w213]
          tunnel: [_ w212] -> w187
          frame False {
          }
          frame True {
            n66 = Add(x=w213, y="跟随偏移 1") -> (x+y=w214:dbl)
            n67 = property on="温控温度 1" class="DigNum (严格)"("Val(Sgnl)"=w214) -> (error out=w212:errorcluster)  [unwired: 2 in, 1 out]
          }
        }
        n68 = case shown="真" w190 {
          tunnel: w206 -> [_ w219]
          tunnel: w187 -> [_ w216]
          frame False {
          }
          frame True {
            n69 = Add(x=w219, y="跟随偏移 2") -> (x+y=w217:dbl)
            n70 = property on="温控温度 2" class="DigNum (严格)"(error in=w216, "Val(Sgnl)"=w217) -> ()  [unwired: 1 in, 2 out]
          }
        }
        n71 = Index Array(array=w197, index #1=1 ("索引"), index #2=2 ("索引"), index #3=3 ("索引"), index #4=4 ("索引"), index #5=5 ("索引"), index #6=6 ("索引"), index #7=7 ("索引"), index #8=8 ("索引")) -> (element #1=w186:dbl, element #2=w185:dbl, element #3=w184:dbl, element #4=w175:dbl, element #5=w174:dbl, element #6=w173:dbl, element #7=w172:dbl, element #8=w171:dbl)
        "实际温度 1" <- w186
        "实际温度 2" <- w174
        n72 = Bundle By Name(cluster=w194, "Time and Data"=w196, "温控情况.实际温度 1"=w186, "输出参数.输出状态 1.实际输出电压"=w185, "输出参数.输出状态 1.实际输出电流"=w184, "输出参数.输出状态 1.实际输出功率"=w175, "温控情况.实际温度 2"=w174, "输出参数.输出状态 2.实际输出电压"=w173, "输出参数.输出状态 2.实际输出电流"=w172, "输出参数.输出状态 2.实际输出功率"=w171) -> (w195:T16)
        n73 = local read "输出状态 1"() -> (w198:T3)
        n74 = Bundle By Name(cluster=w198, "功率输出"=w193, "实际输出电压"=w185, "实际输出电流"=w184) -> (→"输出状态 1":T3)
        n75 = local read "输出状态 2"() -> (w200:T3)
        n76 = Bundle By Name(cluster=w200, "功率输出"=w192, "实际输出电压"=w173, "实际输出电流"=w172) -> (→"输出状态 2":T3)
        n77 = call <vilib>:"Add State(s) to Queue__JKI_lib_State_Machine.vi"("State(s) in Front (\"\")"="UI: Update Graph" ("State(s) in Front (\"\")"), "State(s) in (\"\")"=w210) -> ("States Out"=w211:string)  [unwired: 13 in]
      }
      frame "Data: Cleanup" {
        # "#CSM \"Data: Cleanup\"\nCleanup any data and references, here.\n(this is called automatically, by the Macro: Exit)"
        n78 = Unbundle By Name(w222) -> ("Core.Current VI Reference"=w225:refnum<vi>, "基本信息"=w221:T20)
        n79 = call "CSM - Write Configuration Variable.vim"("Section Name (\"\" as Default)"=w220, "Configuration"=w221) -> ()  [unwired: 6 in, 2 out]
        n80 = Close Reference(reference=w225, error in (no error)=w224) -> (error out=w223:errorcluster)
        n81 = call <vilib>:"Add State(s) to Queue__JKI_lib_State_Machine.vi"("State(s) in (\"\")"=w227) -> ("States Out"=w226:string)  [unwired: 14 in]
      }
      frame "---------- UI ----------" {
        n82 = call <vilib>:"Add State(s) to Queue__JKI_lib_State_Machine.vi"("State(s) in (\"\")"=w229) -> ("States Out"=w228:string)  [unwired: 14 in]
      }
      frame "UI: Initialize" {
        w242 = FALSE ("结束")
        w244 = TRUE
        w243 = T21."Disabled and Grayed Out" ("禁用")
        w248 = waveform(dbl)[][] [] ("历史数据")
        w247 = waveform(dbl)[][] [] ("历史数据")
        n83 = property on="TC1" class="WFChart (严格)"("History Data"=w247) -> ()  [unwired: 2 in, 2 out]
        n84 = property on="TC2" class="WFChart (严格)"("History Data"=w247) -> ()  [unwired: 2 in, 2 out]
        n85 = property on="Power 1" class="WFChart (严格)"("History Data"=w248) -> ()  [unwired: 2 in, 2 out]
        n86 = property on="Power 2" class="WFChart (严格)"("History Data"=w248) -> ()  [unwired: 2 in, 2 out]
        n87 = property on="温控开关 总" class="Bool (严格)"("DisabledEnum"=w243) -> ()  [unwired: 2 in, 2 out]
        n88 = property on="温控开关 1" class="Bool (严格)"("DisabledEnum"=w243) -> ()  [unwired: 2 in, 2 out]
        n89 = property on="温控开关 2" class="Bool (严格)"("DisabledEnum"=w243) -> ()  [unwired: 2 in, 2 out]
        n90 = property on="温控温度 1" class="DigNum (严格)"("DisabledEnum"=w243) -> ()  [unwired: 2 in, 2 out]
        n91 = property on="温控温度 2" class="DigNum (严格)"("DisabledEnum"=w243) -> ()  [unwired: 2 in, 2 out]
        n92 = property on="输出设置 1" class="Clust (严格)"("DisabledEnum"=w243) -> ()  [unwired: 2 in, 2 out]
        n93 = property on="输出设置 2" class="Clust (严格)"("DisabledEnum"=w243) -> ()  [unwired: 2 in, 2 out]
        n94 = property on="PID 2" class="Clust (严格)"("DisabledEnum"=w243) -> ()  [unwired: 2 in, 2 out]
        n95 = property on="PID 1" class="Clust (严格)"("DisabledEnum"=w243) -> ()  [unwired: 2 in, 2 out]
        n96 = property on="过温 1" class="Clust (严格)"("DisabledEnum"=w243) -> ()  [unwired: 2 in, 2 out]
        n97 = property on="过温 2" class="Clust (严格)"("DisabledEnum"=w243) -> ()  [unwired: 2 in, 2 out]
        n98 = property on="过压/过流 1" class="Clust (严格)"("DisabledEnum"=w243) -> ()  [unwired: 2 in, 2 out]
        n99 = property on="过压/过流 2" class="Clust (严格)"("DisabledEnum"=w243) -> ()  [unwired: 2 in, 2 out]
        n100 = property on="保护结果 1" class="Clust (严格)"("DisabledEnum"=w243) -> ()  [unwired: 2 in, 2 out]
        n101 = property on="保护结果 2" class="Clust (严格)"("DisabledEnum"=w243) -> ()  [unwired: 2 in, 2 out]
        n102 = property on="温控循环功能开启" class="Bool (严格)"("DisabledEnum"=w243) -> ()  [unwired: 2 in, 2 out]
        n103 = Unbundle By Name(w245) -> ("温控情况.温控温度 1"=w238:dbl, "温控情况.温控温度 2"=w237:dbl, "温控情况.打开串口"=w241:bool, "开关信息.开关 1"=w240:bool, "开关信息.开关 2"=w239:bool, "基本信息"=w236:T20, "子程序.子程序？"=w233:bool)
        n104 = Unbundle By Name(w236) -> ("USB Port"=w235:refnum<visa-resource-name>, "采集间隔(s)"=w234:dbl)
        n105 = local write "温控循环功能开启"(w242) -> ()
        n106 = local write "Fast Mode"(w242) -> ()
        n107 = local write "温控-错误输出"(errorcluster {"status"=FALSE, "code"=0, "source"=""} ("Error Out")) -> ()
        n108 = local write "通道"(w244) -> ()
        n109 = local write "温度"(w244) -> ()
        n110 = Not(x=w233) -> (.not. x?=w232:bool)
        n111 = local write "温控温度 1"(w238) -> ()
        n112 = local write "温控温度 2"(w237) -> ()
        n113 = local write "打开串口"(w241) -> ()
        n114 = local write "温控开关 1"(w240) -> ()
        n115 = local write "温控开关 2"(w239) -> ()
        n116 = local write "温控串口"(w235) -> ()
        n117 = local write "采集间隔"(w234) -> ()
        n118 = property on="停止" class="Bool"("Visible"=w232) -> ()  [unwired: 2 in, 2 out]
        n119 = call <vilib>:"Add State(s) to Queue__JKI_lib_State_Machine.vi"("State(s) in (\"\")"=w250) -> ("States Out"=w249:string)  [unwired: 14 in]
      }
      frame "UI: Start" {
        w254 = T21."Enabled" ("禁用")
        n120 = Unbundle By Name(w256) -> ("设备信息.双通道设备？"=w255:bool)
        n121 = property on="保护结果 1" class="Clust (严格)"("DisabledEnum"=w254) -> ()  [unwired: 2 in, 2 out]
        n122 = property on="温控循环功能开启" class="Bool (严格)"("DisabledEnum"=w254) -> ()  [unwired: 2 in, 2 out]
        n123 = property on="温控开关 1" class="Bool (严格)"("DisabledEnum"=w254) -> ()  [unwired: 2 in, 2 out]
        n124 = property on="温控温度 1" class="DigNum (严格)"("DisabledEnum"=w254) -> ()  [unwired: 2 in, 2 out]
        n125 = property on="输出设置 1" class="Clust (严格)"("DisabledEnum"=w254) -> ()  [unwired: 2 in, 2 out]
        n126 = property on="PID 1" class="Clust (严格)"("DisabledEnum"=w254) -> ()  [unwired: 2 in, 2 out]
        n127 = property on="过温 1" class="Clust (严格)"("DisabledEnum"=w254) -> ()  [unwired: 2 in, 2 out]
        n128 = property on="过压/过流 1" class="Clust (严格)"("DisabledEnum"=w254) -> ()  [unwired: 2 in, 2 out]
        n129 = case shown="真" w255 {
          tunnel: w254 -> [_ w259]
          tunnel: w254 -> [_ w258]
          frame False {
          }
          frame True {
            n130 = property on="温控开关 2" class="Bool (严格)"("DisabledEnum"=w259) -> ()  [unwired: 2 in, 2 out]
            n131 = property on="温控温度 2" class="DigNum (严格)"("DisabledEnum"=w259) -> ()  [unwired: 2 in, 2 out]
            n132 = property on="输出设置 2" class="Clust (严格)"("DisabledEnum"=w259) -> ()  [unwired: 2 in, 2 out]
            n133 = property on="PID 2" class="Clust (严格)"("DisabledEnum"=w259) -> ()  [unwired: 2 in, 2 out]
            n134 = property on="过温 2" class="Clust (严格)"("DisabledEnum"=w259) -> ()  [unwired: 2 in, 2 out]
            n135 = property on="过压/过流 2" class="Clust (严格)"("DisabledEnum"=w259) -> ()  [unwired: 2 in, 2 out]
            n136 = property on="保护结果 2" class="Clust (严格)"("DisabledEnum"=w259) -> ()  [unwired: 2 in, 2 out]
            n137 = property on="温控开关 总" class="Bool (严格)"("DisabledEnum"=w258) -> ()  [unwired: 2 in, 2 out]
          }
        }
        n138 = call <vilib>:"Add State(s) to Queue__JKI_lib_State_Machine.vi"("State(s) in (\"\")"=w252) -> ("States Out"=w253:string)  [unwired: 14 in]
      }
      frame "UI: Output1" {
        # "输出模式"
        # "最大输出电压"
        n139 = Unbundle By Name(w275) -> ("基本信息.USB Port"=w274:refnum<visa-resource-name>)
        n140 = call "串口读写 - WK.vi"("错误输入（无错误）"=w273, "写入设备"="TC1:TCADJUSTTEMP?\r" ("写入缓冲区"), "VISA输入"=w274) -> ("错误输出"=w282:errorcluster, "读取设备(n)"=w281:dbl, "VISA输出"=w283:refnum<visa-resource-name>)  [unwired: 5 in, 1 out]
        n141 = local write "温控温度 1"(w281) -> ()
        n142 = call "串口读写 - WK.vi"("错误输入（无错误）"=w282, "写入设备"="TC1:TCSW?\r" ("写入缓冲区"), "VISA输入"=w283) -> ("错误输出"=w264:errorcluster, "读取设备(n)"=w260:dbl, "VISA输出"=w265:refnum<visa-resource-name>)  [unwired: 5 in, 1 out]
        n143 = Not Equal To 0?(x=w260) -> (x != 0?=w278:bool)
        n144 = local read "输出状态 1"() -> (w280:T3)
        n145 = local write "温控开关 1"(w278) -> ()
        n146 = Bundle By Name(cluster=w280, "功率输出"=w260) -> (w279:T3)
        n147 = local write "输出状态 1"(w279) -> ()
        n148 = call "串口读写 - WK.vi"("错误输入（无错误）"=w264, "写入设备"="TC1:TCMAXV?\r" ("写入缓冲区"), "VISA输入"=w265) -> ("错误输出"=w269:errorcluster, "读取设备(n)"=w268:dbl, "VISA输出"=w272:refnum<visa-resource-name>)  [unwired: 5 in, 1 out]
        n149 = call "串口读写 - WK.vi"("错误输入（无错误）"=w269, "写入设备"="TC1:TCMODE?\r" ("写入缓冲区"), "VISA输入"=w272) -> ("错误输出"=w263:errorcluster, "读取设备(n)"=w270:dbl)  [unwired: 5 in, 2 out]
        n150 = local read "输出设置 1"() -> (w271:T4)
        n151 = Bundle By Name(cluster=w271, "输出模式"=w270, "最大输出电压"=w268) -> (w262:T4)
        n152 = local write "输出设置 1"(w262) -> ()
        n153 = Bundle By Name(cluster=w275, "温控情况.温控温度 1"=w281, "开关信息.开关 1"=w278, "输出参数.输出状态 1.功率输出"=w260, "输出参数.输出设置 1"=w262) -> (w261:T16)
        n154 = call <vilib>:"Add State(s) to Queue__JKI_lib_State_Machine.vi"("State(s) in (\"\")"=w284) -> ("States Out"=w285:string)  [unwired: 14 in]
      }
      frame "UI: Output2" {
        n155 = Unbundle By Name(w303) -> ("基本信息.USB Port"=w304:refnum<visa-resource-name>)
        n156 = call "串口读写 - WK.vi"("错误输入（无错误）"=w288, "写入设备"="TC2:TCADJUSTTEMP?\r" ("写入缓冲区"), "VISA输入"=w304) -> ("错误输出"=w307:errorcluster, "读取设备(n)"=w289:dbl, "VISA输出"=w308:refnum<visa-resource-name>)  [unwired: 5 in, 1 out]
        n157 = local write "温控温度 2"(w289) -> ()
        n158 = call "串口读写 - WK.vi"("错误输入（无错误）"=w307, "写入设备"="TC2:TCSW?\r" ("写入缓冲区"), "VISA输入"=w308) -> ("错误输出"=w293:errorcluster, "读取设备(n)"=w286:dbl, "VISA输出"=w294:refnum<visa-resource-name>)  [unwired: 5 in, 1 out]
        n159 = Not Equal To 0?(x=w286) -> (x != 0?=w290:bool)
        n160 = local write "温控开关 2"(w290) -> ()
        n161 = local read "输出状态 2"() -> (w309:T3)
        n162 = Bundle By Name(cluster=w309, "功率输出"=w286) -> (w291:T3)
        n163 = local write "输出状态 2"(w291) -> ()
        n164 = call "串口读写 - WK.vi"("错误输入（无错误）"=w293, "写入设备"="TC2:TCMAXV?\r" ("写入缓冲区"), "VISA输入"=w294) -> ("错误输出"=w300:errorcluster, "读取设备(n)"=w301:dbl, "VISA输出"=w297:refnum<visa-resource-name>)  [unwired: 5 in, 1 out]
        n165 = local read "输出设置 2"() -> (w299:T4)
        n166 = call "串口读写 - WK.vi"("错误输入（无错误）"=w300, "写入设备"="TC2:TCMODE?\r" ("写入缓冲区"), "VISA输入"=w297) -> ("错误输出"=w287:errorcluster, "读取设备(n)"=w298:dbl)  [unwired: 5 in, 2 out]
        n167 = Bundle By Name(cluster=w299, "输出模式"=w298, "最大输出电压"=w301) -> (w292:T4)
        n168 = local write "输出设置 2"(w292) -> ()
        n169 = Bundle By Name(cluster=w303, "温控情况.温控温度 2"=w289, "开关信息.开关 2"=w290, "输出参数.输出状态 2.功率输出"=w286, "输出参数.输出设置 2"=w292) -> (w302:T16)
        n170 = call <vilib>:"Add State(s) to Queue__JKI_lib_State_Machine.vi"("State(s) in (\"\")"=w310) -> ("States Out"=w311:string)  [unwired: 14 in]
      }
      frame "UI: PID1" {
        # "控制间隔"
        # "D值"
        # "I值"
        # "P值"
        # "PID类型"
        n171 = Unbundle By Name(w315) -> ("基本信息.USB Port"=w317:refnum<visa-resource-name>)
        n172 = call "串口读写 - WK.vi"("错误输入（无错误）"=w313, "写入设备"="TC1:TCPIDTYPE?\r" ("写入缓冲区"), "VISA输入"=w317) -> ("错误输出"=w336:errorcluster, "读取设备(n)"=w328:dbl, "VISA输出"=w340:refnum<visa-resource-name>)  [unwired: 5 in, 1 out]
        n173 = call "串口读写 - WK.vi"("错误输入（无错误）"=w336, "写入设备"="TC1:TCP?\r" ("写入缓冲区"), "VISA输入"=w340) -> ("错误输出"=w335:errorcluster, "读取设备(n)"=w329:dbl, "VISA输出"=w339:refnum<visa-resource-name>)  [unwired: 5 in, 1 out]
        n174 = call "串口读写 - WK.vi"("错误输入（无错误）"=w335, "写入设备"="TC1:TCTI?\r" ("写入缓冲区"), "VISA输入"=w339) -> ("错误输出"=w334:errorcluster, "读取设备(n)"=w330:dbl, "VISA输出"=w338:refnum<visa-resource-name>)  [unwired: 5 in, 1 out]
        n175 = call "串口读写 - WK.vi"("错误输入（无错误）"=w334, "写入设备"="TC1:TCTD?\r" ("写入缓冲区"), "VISA输入"=w338) -> ("错误输出"=w333:errorcluster, "读取设备(n)"=w331:dbl, "VISA输出"=w337:refnum<visa-resource-name>)  [unwired: 5 in, 1 out]
        n176 = call "串口读写 - WK.vi"("错误输入（无错误）"=w333, "写入设备"="TC1:TCCTRLINTERVAL?\r" ("写入缓冲区"), "VISA输入"=w337) -> ("错误输出"=w325:errorcluster, "读取设备(n)"=w327:dbl, "VISA输出"=w326:refnum<visa-resource-name>)  [unwired: 5 in, 1 out]
        n177 = call "串口读写 - WK.vi"("错误输入（无错误）"=w325, "写入设备"="TC1:TCPIDCAL?\r" ("写入缓冲区"), "VISA输入"=w326) -> ("错误输出"=w312:errorcluster, "读取设备(n)"=w324:dbl)  [unwired: 5 in, 2 out]
        n178 = local read "PID 1"() -> (w332:T5)
        n179 = Bundle By Name(cluster=w332, "PID类型"=w328, "P"=w329, "I"=w330, "D"=w331, "PID控制间隔"=w327, "PID计算方法"=w324) -> (w316:T5)
        n180 = local write "PID 1"(w316) -> ()
        n181 = Bundle By Name(cluster=w315, "输出参数.PID 1"=w316) -> (w314:T16)
        n182 = call <vilib>:"Add State(s) to Queue__JKI_lib_State_Machine.vi"("State(s) in (\"\")"=w341) -> ("States Out"=w342:string)  [unwired: 14 in]
      }
      frame "UI: PID2" {
        # "控制间隔"
        # "D值"
        # "I值"
        # "P值"
        # "PID类型"
        n183 = Unbundle By Name(w346) -> ("基本信息.USB Port"=w345:refnum<visa-resource-name>)
        n184 = call "串口读写 - WK.vi"("错误输入（无错误）"=w344, "写入设备"="TC2:TCPIDTYPE?\r" ("写入缓冲区"), "VISA输入"=w345) -> ("错误输出"=w358:errorcluster, "读取设备(n)"=w363:dbl, "VISA输出"=w354:refnum<visa-resource-name>)  [unwired: 5 in, 1 out]
        n185 = call "串口读写 - WK.vi"("错误输入（无错误）"=w358, "写入设备"="TC2:TCP?\r" ("写入缓冲区"), "VISA输入"=w354) -> ("错误输出"=w359:errorcluster, "读取设备(n)"=w364:dbl, "VISA输出"=w355:refnum<visa-resource-name>)  [unwired: 5 in, 1 out]
        n186 = call "串口读写 - WK.vi"("错误输入（无错误）"=w359, "写入设备"="TC2:TCTI?\r" ("写入缓冲区"), "VISA输入"=w355) -> ("错误输出"=w360:errorcluster, "读取设备(n)"=w365:dbl, "VISA输出"=w356:refnum<visa-resource-name>)  [unwired: 5 in, 1 out]
        n187 = call "串口读写 - WK.vi"("错误输入（无错误）"=w360, "写入设备"="TC2:TCTD?\r" ("写入缓冲区"), "VISA输入"=w356) -> ("错误输出"=w361:errorcluster, "读取设备(n)"=w366:dbl, "VISA输出"=w357:refnum<visa-resource-name>)  [unwired: 5 in, 1 out]
        n188 = call "串口读写 - WK.vi"("错误输入（无错误）"=w361, "写入设备"="TC2:TCCTRLINTERVAL?\r" ("写入缓冲区"), "VISA输入"=w357) -> ("错误输出"=w369:errorcluster, "读取设备(n)"=w367:dbl, "VISA输出"=w368:refnum<visa-resource-name>)  [unwired: 5 in, 1 out]
        n189 = call "串口读写 - WK.vi"("错误输入（无错误）"=w369, "写入设备"="TC2:TCPIDCAL?\r" ("写入缓冲区"), "VISA输入"=w368) -> ("错误输出"=w343:errorcluster, "读取设备(n)"=w370:dbl)  [unwired: 5 in, 2 out]
        n190 = local read "PID 2"() -> (w362:T5)
        n191 = Bundle By Name(cluster=w362, "PID类型"=w363, "P"=w364, "I"=w365, "D"=w366, "PID控制间隔"=w367, "PID计算方法"=w370) -> (w347:T5)
        n192 = local write "PID 2"(w347) -> ()
        n193 = call <vilib>:"Add State(s) to Queue__JKI_lib_State_Machine.vi"("State(s) in (\"\")"=w372) -> ("States Out"=w373:string)  [unwired: 14 in]
        n194 = Bundle By Name(cluster=w346, "输出参数.PID 2"=w347) -> (w371:T16)
      }
      frame "UI: Protect1" {
        # "温度限速"
        # "最高设定温度"
        # "最低设定温度"
        # "过温保护高阈值"
        # "过温保护低阈值"
        # "过温保护开关"
        # "过温保护结果"
        # "过流保护结果"
        # "过压保护结果"
        # "过流保护"
        # "过压保护"
        n195 = Unbundle By Name(w406) -> ("设备信息.设备型号"=w422:string, "基本信息.USB Port"=w428:refnum<visa-resource-name>)
        n196 = Equal?(x="TCM1040\r" ("y"), y=w422) -> (x = y?=w407:bool)
        n197 = call "串口读写 - WK.vi"("错误输入（无错误）"=w376, "写入设备"="TC1:TCADJUSTOVPV?\r" ("写入缓冲区"), "VISA输入"=w428) -> ("错误输出"=w426:errorcluster, "读取设备(n)"=w424:dbl, "VISA输出"=w427:refnum<visa-resource-name>)  [unwired: 5 in, 1 out]
        n198 = case shown="假" w407 {
          tunnel: w427 -> [w444 w447]
          tunnel: [w443 w447] -> w409
          tunnel: [w442 w448] -> w408
          tunnel: w426 -> [w441 w448]
          tunnel: [w440 2.0 ("读取设备(n)")] -> w423
          frame False {
            n199 = call "串口读写 - WK.vi"("错误输入（无错误）"=w441, "写入设备"="TC1:TCADJUSTOCPC?\r" ("写入缓冲区"), "VISA输入"=w444) -> ("错误输出"=w442:errorcluster, "读取设备(n)"=w440:dbl, "VISA输出"=w443:refnum<visa-resource-name>)  [unwired: 5 in, 1 out]
          }
          frame True {
          }
        }
        n200 = local read "过压/过流 1"() -> (w425:cluster{"过压保护阈值":dbl, "过流保护阈值":dbl})
        n201 = Bundle By Name(cluster=w425, "过压保护阈值"=w424, "过流保护阈值"=w423) -> (w405:cluster{"过压保护阈值":dbl, "过流保护阈值":dbl})
        n202 = local write "过压/过流 1"(w405) -> ()
        n203 = call "串口读写 - WK.vi"("错误输入（无错误）"=w408, "写入设备"="TC1:TCOVEF?\r" ("写入缓冲区"), "VISA输入"=w409) -> ("错误输出"=w417:errorcluster, "读取设备(n)"=w414:dbl, "VISA输出"=w419:refnum<visa-resource-name>)  [unwired: 5 in, 1 out]
        n204 = case shown="假" w407 {
          tunnel: w419 -> [w435 w439]
          tunnel: [w434 w439] -> w418
          tunnel: w417 -> [w433 w438]
          tunnel: [w432 w438] -> w416
          tunnel: [w431 1.0 ("读取设备(n)")] -> w413
          frame False {
            n205 = call "串口读写 - WK.vi"("错误输入（无错误）"=w433, "写入设备"="TC1:TCOCEF?\r" ("写入缓冲区"), "VISA输入"=w435) -> ("错误输出"=w432:errorcluster, "读取设备(n)"=w431:dbl, "VISA输出"=w434:refnum<visa-resource-name>)  [unwired: 5 in, 1 out]
          }
          frame True {
          }
        }
        n206 = call "串口读写 - WK.vi"("错误输入（无错误）"=w416, "写入设备"="TC1:TCOTEF?\r" ("写入缓冲区"), "VISA输入"=w418) -> ("错误输出"=w378:errorcluster, "读取设备(n)"=w412:dbl, "VISA输出"=w379:refnum<visa-resource-name>)  [unwired: 5 in, 1 out]
        n207 = call "串口读写 - WK.vi"("错误输入（无错误）"=w378, "写入设备"="TC1:TCOTPE?\r" ("写入缓冲区"), "VISA输入"=w379) -> ("错误输出"=w399:errorcluster, "读取设备(n)"=w394:dbl, "VISA输出"=w403:refnum<visa-resource-name>)  [unwired: 5 in, 1 out]
        n208 = Not Equal To 0?(x=w394) -> (x != 0?=w393:bool)
        n209 = call "串口读写 - WK.vi"("错误输入（无错误）"=w399, "写入设备"="TC1:TCOTPLT?\r" ("写入缓冲区"), "VISA输入"=w403) -> ("错误输出"=w398:errorcluster, "读取设备(n)"=w392:dbl, "VISA输出"=w402:refnum<visa-resource-name>)  [unwired: 5 in, 1 out]
        n210 = call "串口读写 - WK.vi"("错误输入（无错误）"=w398, "写入设备"="TC1:TCOTPHT?\r" ("写入缓冲区"), "VISA输入"=w402) -> ("错误输出"=w397:errorcluster, "读取设备(n)"=w391:dbl, "VISA输出"=w401:refnum<visa-resource-name>)  [unwired: 5 in, 1 out]
        n211 = call "串口读写 - WK.vi"("错误输入（无错误）"=w397, "写入设备"="TC1:TCMINSETTEMP?\r" ("写入缓冲区"), "VISA输入"=w401) -> ("错误输出"=w396:errorcluster, "读取设备(n)"=w390:dbl, "VISA输出"=w400:refnum<visa-resource-name>)  [unwired: 5 in, 1 out]
        n212 = call "串口读写 - WK.vi"("错误输入（无错误）"=w396, "写入设备"="TC1:TCMAXSETTEMP?\r" ("写入缓冲区"), "VISA输入"=w400) -> ("错误输出"=w387:errorcluster, "读取设备(n)"=w389:dbl, "VISA输出"=w388:refnum<visa-resource-name>)  [unwired: 5 in, 1 out]
        n213 = call "串口读写 - WK.vi"("错误输入（无错误）"=w387, "写入设备"="TC1:TCRAMPSPEED?\r" ("写入缓冲区"), "VISA输入"=w388) -> ("错误输出"=w375:errorcluster, "读取设备(n)"=w386:dbl)  [unwired: 5 in, 2 out]
        n214 = local read "过温 1"() -> (w395:T6)
        n215 = local read "保护结果 1"() -> (w415:T7)
        n216 = Bundle By Name(cluster=w395, "过温保护开关"=w393, "过温保护低阈值"=w392, "过温保护高阈值"=w391, "最低设定温度"=w390, "最高设定温度"=w389, "温度限速"=w386) -> (w377:T6)
        n217 = Bundle By Name(cluster=w415, "过压保护结果"=w414, "过流保护结果"=w413, "过温保护结果"=w412) -> (w374:T7)
        "保护结果 1" <- w374
        n218 = local write "过温 1"(w377) -> ()
        n219 = call <vilib>:"Add State(s) to Queue__JKI_lib_State_Machine.vi"("State(s) in (\"\")"=w429) -> ("States Out"=w430:string)  [unwired: 14 in]
        n220 = Bundle By Name(cluster=w406, "保护.过压/过流 1"=w405, "保护.保护结果 1"=w374, "保护.过温 1"=w377) -> (w404:T16)
      }
      frame "UI: Protect2" {
        # "温度限速"
        # "最高设定温度"
        # "最低设定温度"
        # "过温保护高阈值"
        # "过温保护低阈值"
        # "过温保护开关"
        # "过流保护"
        # "过压保护"
        # "过温保护结果"
        # "过流保护结果"
        # "过压保护结果"
        n221 = Unbundle By Name(w484) -> ("基本信息.USB Port"=w482:refnum<visa-resource-name>)
        n222 = call "串口读写 - WK.vi"("错误输入（无错误）"=w451, "写入设备"="TC2:TCADJUSTOVPV?\r" ("写入缓冲区"), "VISA输入"=w482) -> ("错误输出"=w488:errorcluster, "读取设备(n)"=w489:dbl, "VISA输出"=w487:refnum<visa-resource-name>)  [unwired: 5 in, 1 out]
        n223 = call "串口读写 - WK.vi"("错误输入（无错误）"=w488, "写入设备"="TC2:TCADJUSTOCPC?\r" ("写入缓冲区"), "VISA输入"=w487) -> ("错误输出"=w480:errorcluster, "读取设备(n)"=w490:dbl, "VISA输出"=w481:refnum<visa-resource-name>)  [unwired: 5 in, 1 out]
        n224 = local read "过压/过流 2"() -> (w491:cluster{"过压保护阈值":dbl, "过流保护阈值":dbl})
        n225 = Bundle By Name(cluster=w491, "过压保护阈值"=w489, "过流保护阈值"=w490) -> (w479:cluster{"过压保护阈值":dbl, "过流保护阈值":dbl})
        n226 = local write "过压/过流 2"(w479) -> ()
        n227 = call "串口读写 - WK.vi"("错误输入（无错误）"=w480, "写入设备"="TC2:TCOVEF?\r" ("写入缓冲区"), "VISA输入"=w481) -> ("错误输出"=w500:errorcluster, "读取设备(n)"=w498:dbl, "VISA输出"=w502:refnum<visa-resource-name>)  [unwired: 5 in, 1 out]
        n228 = call "串口读写 - WK.vi"("错误输入（无错误）"=w500, "写入设备"="TC2:TCOCEF?\r" ("写入缓冲区"), "VISA输入"=w502) -> ("错误输出"=w499:errorcluster, "读取设备(n)"=w497:dbl, "VISA输出"=w501:refnum<visa-resource-name>)  [unwired: 5 in, 1 out]
        n229 = call "串口读写 - WK.vi"("错误输入（无错误）"=w499, "写入设备"="TC2:TCOTEF?\r" ("写入缓冲区"), "VISA输入"=w501) -> ("错误输出"=w453:errorcluster, "读取设备(n)"=w496:dbl, "VISA输出"=w454:refnum<visa-resource-name>)  [unwired: 5 in, 1 out]
        n230 = call "串口读写 - WK.vi"("错误输入（无错误）"=w453, "写入设备"="TC2:TCOTPE?\r" ("写入缓冲区"), "VISA输入"=w454) -> ("错误输出"=w465:errorcluster, "读取设备(n)"=w469:dbl, "VISA输出"=w461:refnum<visa-resource-name>)  [unwired: 5 in, 1 out]
        n231 = Not Equal To 0?(x=w469) -> (x != 0?=w470:bool)
        n232 = call "串口读写 - WK.vi"("错误输入（无错误）"=w465, "写入设备"="TC2:TCOTPLT?\r" ("写入缓冲区"), "VISA输入"=w461) -> ("错误输出"=w466:errorcluster, "读取设备(n)"=w471:dbl, "VISA输出"=w462:refnum<visa-resource-name>)  [unwired: 5 in, 1 out]
        n233 = call "串口读写 - WK.vi"("错误输入（无错误）"=w466, "写入设备"="TC2:TCOTPHT?\r" ("写入缓冲区"), "VISA输入"=w462) -> ("错误输出"=w467:errorcluster, "读取设备(n)"=w472:dbl, "VISA输出"=w463:refnum<visa-resource-name>)  [unwired: 5 in, 1 out]
        n234 = call "串口读写 - WK.vi"("错误输入（无错误）"=w467, "写入设备"="TC2:TCMINSETTEMP?\r" ("写入缓冲区"), "VISA输入"=w463) -> ("错误输出"=w468:errorcluster, "读取设备(n)"=w473:dbl, "VISA输出"=w464:refnum<visa-resource-name>)  [unwired: 5 in, 1 out]
        n235 = call "串口读写 - WK.vi"("错误输入（无错误）"=w468, "写入设备"="TC2:TCMAXSETTEMP?\r" ("写入缓冲区"), "VISA输入"=w464) -> ("错误输出"=w476:errorcluster, "读取设备(n)"=w474:dbl, "VISA输出"=w475:refnum<visa-resource-name>)  [unwired: 5 in, 1 out]
        n236 = call "串口读写 - WK.vi"("错误输入（无错误）"=w476, "写入设备"="TC2:TCRAMPSPEED?\r" ("写入缓冲区"), "VISA输入"=w475) -> ("错误输出"=w450:errorcluster, "读取设备(n)"=w477:dbl)  [unwired: 5 in, 2 out]
        n237 = local read "保护结果 2"() -> (w495:T7)
        n238 = Bundle By Name(cluster=w495, "过压保护结果"=w498, "过流保护结果"=w497, "过温保护结果"=w496) -> (w449:T7)
        "保护结果 2" <- w449
        n239 = local read "过温 2"() -> (w478:T6)
        n240 = Bundle By Name(cluster=w478, "过温保护开关"=w470, "过温保护低阈值"=w471, "过温保护高阈值"=w472, "最低设定温度"=w473, "最高设定温度"=w474, "温度限速"=w477) -> (w452:T6)
        n241 = local write "过温 2"(w452) -> ()
        n242 = call <vilib>:"Add State(s) to Queue__JKI_lib_State_Machine.vi"("State(s) in (\"\")"=w503) -> ("States Out"=w504:string)  [unwired: 14 in]
        n243 = Bundle By Name(cluster=w484, "保护.过压/过流 2"=w479, "保护.保护结果 2"=w449, "保护.过温 2"=w452) -> (w483:T16)
      }
      frame "UI: Update Graph" {
        n244 = Unbundle By Name(w507) -> ("温控情况.温控温度 1"=w525:dbl, "温控情况.实际温度 1"=w526:dbl, "温控情况.温控温度 2"=w524:dbl, "温控情况.实际温度 2"=w523:dbl, "Time and Data.采集时间"=w518:timestamp, "输出参数.输出状态 1.实际输出功率"=w506:dbl, "输出参数.输出状态 2.实际输出功率"=w505:dbl, "基本信息.采集间隔(s)"=w517:dbl, "开关信息.开关 1"=w516:bool, "开关信息.开关 2"=w515:bool)  [unwired: 2 out]
        n245 = local write "温控开关 1"(w516) -> ()
        n246 = local write "温控开关 2"(w515) -> ()
        n247 = Build Array(w525) -> (w531:dbl[])
        n248 = Build Array(w506) -> (w519:dbl[])
        n249 = Build Array(w524) -> (w530:dbl[])
        n250 = Build Array(w505) -> (w520:dbl[])
        n251 = Build Array(w526) -> (w528:dbl[])
        n252 = Build Array(w523) -> (w529:dbl[])
        n253 = Bundle By Name("Y"=w519, "t0"=w518, "dt"=w517) -> (w514:waveform(dbl))  [unwired: 1 in]
        n254 = Bundle By Name("Y"=w531, "t0"=w518, "dt"=w517) -> (w510:waveform(dbl))  [unwired: 1 in]
        n255 = Bundle By Name("Y"=w530, "t0"=w518, "dt"=w517) -> (w508:waveform(dbl))  [unwired: 1 in]
        n256 = Bundle By Name("Y"=w520, "t0"=w518, "dt"=w517) -> (w509:waveform(dbl))  [unwired: 1 in]
        n257 = Bundle By Name("Y"=w528, "t0"=w518, "dt"=w517) -> (w512:waveform(dbl))  [unwired: 1 in]
        n258 = Bundle By Name("Y"=w529, "t0"=w518, "dt"=w517) -> (w527:waveform(dbl))  [unwired: 1 in]
        n259 = Build Array(w509, w508) -> (→"Power 2":waveform(dbl)[])
        n260 = Build Array(w508, w527) -> (→"TC2":waveform(dbl)[])
        n261 = Build Array(w514, w510) -> (→"Power 1":waveform(dbl)[])
        n262 = Build Array(w510, w512) -> (→"TC1":waveform(dbl)[])
        n263 = call <vilib>:"Add State(s) to Queue__JKI_lib_State_Machine.vi"("State(s) in (\"\")"=w533) -> ("States Out"=w532:string)  [unwired: 14 in]
      }
      frame "---------- Macro ----------" {
        # "#CSM \"Category Seperator\"\nDo not put any code in this frame."
        n264 = call <vilib>:"Add State(s) to Queue__JKI_lib_State_Machine.vi"("State(s) in (\"\")"=w537) -> ("States Out"=w536:string)  [unwired: 14 in]
      }
      frame "Macro: Initialize" {
        w540 = "Data: Initialize\nInitialize Core Data\nData: Update Indicators\n\nUI: Initialize\n\n//Permanent registrations\nAcquired Data@Acquisition - <1> >> Data: Update Indicators -><register>\nAcquired Data@Acquisition - <1> >> API: Log@Logging - <1> -><register>\n\n//Error registrations\nError Occurred@Acquisition - <1> >> Error Handler -><register>\nError Occurred@Logging - <1> >> Error Handler -><register>\n\n//Dynamic registrations\n// 订阅/取消订阅\n//Status@SourceModule >> API@TargetModule -><register as interrupt>\n//UrgentEvent @SourceModule >> API@TargetModule -><register as status>"  # Data: Initialize Initialize Core Data Data: Update Indicators  UI: Initialize  //Permanent registrations Acquired Data@Acquisition - <1> >> Data: Update Indicators -><register> Acquired Data@Acquisition - <1> >> API: Log@Logging - <1> -><register>  //Error registrations Error Occurred@Acquisition - <1> >> Error Handler -><register> Error Occurred@Logging - <1> >> Error Handler -><register>  //Dynamic registrations // 订阅/取消订阅 //Status@SourceModule >> API@TargetModule -><register as interrupt> //UrgentEvent @SourceModule >> API@TargetModule -><register as status>
        # "#CSM \"Macro: Initialize\"\nInitialization Macro (This is called once, when the VI starts)"
        n265 = call-poly <userlib>:"Build Message with Arguments++.vi"("States With Replace Token"=w540, "<1>"=w539) -> ("States"=w538:string)  [unwired: 13 in]
        n266 = call <vilib>:"Add State(s) to Queue__JKI_lib_State_Machine.vi"("State(s) in Front (\"\")"=w538, "State(s) in (\"\")"=w543) -> ("States Out"=w542:string)  [unwired: 13 in]
      }
      frame "Macro: Start" {
        n267 = Unbundle By Name(T12 {"波特率"=57600, "数据位"=8, "校验"=enum."None", "停止位"=10, "流控制"=0} ("串口设置")) -> ("波特率"=w584:u32, "数据位"=w583:u16, "校验"=w582:enum16{"None", "Odd", "Even", "Mark", "Space"}, "停止位"=w585:u16, "流控制"=w586:u16)
        n268 = call-poly "VISA Configure Serial Port"("VISA resource name"="温控串口", "baud rate (9600)"=w584, "data bits (8)"=w583, "parity (0:none)"=w582, "stop bits (10: 1 bit)"=w585, "flow control (0:none)"=w586) -> ("VISA resource name out"=w580:refnum<visa-resource-name>, "error out"=w578:errorcluster)  [unwired: 3 in, 5 out]
        n269 = Concatenate Strings("MEMORY:MEMWP=" ("写入缓冲区"), "0" ("字符串"), "\r" ("写入缓冲区")) -> (w581:string)
        n270 = local read "采集间隔"() -> (w550:dbl)
        n271 = call "串口读写 - WK.vi"("错误输入（无错误）"=w578, "写入设备"=w581, "VISA输入"=w580) -> ("错误输出"=w577:errorcluster, "VISA输出"=w579:refnum<visa-resource-name>)  [unwired: 5 in, 2 out]
        n272 = call "串口读写 - WK.vi"("错误输入（无错误）"=w577, "写入设备"="SYSTEM:SYSMODEL?\r" ("写入缓冲区"), "VISA输入"=w579) -> ("读取设备"=w565:string)  [unwired: 5 in, 3 out]
        "温控器设备型号" <- w565
        n273 = Not Equal?(x=w565, y="TCM1031\r") -> (x != y?=w576:bool)
        n274 = Not Equal?(x=w565, y="TCM1040\r") -> (x != y?=w575:bool)
        n275 = Compound Arithmetic op=AND(w576, w575) -> (w554:bool)
        n276 = Bundle By Name(cluster=w567, "基本信息.USB Port"="温控串口", "基本信息.采集间隔(s)"=w550, "设备信息.设备型号"=w565, "设备信息.双通道设备？"=w554, "温控情况.打开串口"=TRUE) -> (w561:T16)
        n277 = Unbundle By Name(w561) -> ("基本信息"=w548:T20, "设备信息"=w560:cluster{"设备型号":string, "双通道设备？":bool}, "开关信息"=w552:cluster{"开关 1":bool, "开关 2":bool, "温控是否打开":bool}, "温控情况.温控温度 1"=w546:dbl, "温控情况.温控温度 2"=w545:dbl)
        n278 = Bundle("温控温度 1"=w546, "温控温度 2"=w545) -> (w544:cluster{"温控温度 1":dbl, "温控温度 2":dbl})  [unwired: 1 in]
        n279 = Bundle(cluster=T11 {"基本信息"={"USB Port"="", "采集间隔(s)"=0.0}, "设备信息"={"设备型号"="", "双通道设备？"=FALSE}, "开关"={"开关 1"=FALSE, "开关 2"=FALSE, "Fast Mode"=FALSE}, "Control Temp"={"Control Temp 1"=0.0, "Control Temp 2"=0.0}} ("Device Info"), "基本信息"=w548, "设备信息"=w560, "开关"=w552, "Control Temp"=w544) -> (w559:T11)
        n280 = Select(t="UI: Output2\nUI: PID2\nUI: Protect2" ("State"), s=w554, f="") -> (s? t:f=w555:string)
        n281 = call "Convert Data To API String Arguments.vim"("Data"=w559) -> ("API String"=w563:string)  [unwired: 7 in, 1 out]
        n282 = call-poly <userlib>:"Build Message with Arguments++.vi"("States With Replace Token"="API: Start >> <param> -@ Acquisition - <1>\nAPI: Start  -@ Logging - <1>\n\nUI: Start\nUI: Output1\nUI: PID1\nUI: Protect1" ("State"), "<param>"=w563, "<1>"=w562) -> ("States"=w558:string)  [unwired: 12 in]
        n283 = call <vilib>:"Add State(s) to Queue__JKI_lib_State_Machine.vi"("State(s) in Front (\"\")"=w558, "State(s) in (\"\")"=w555) -> ("States Out"=w547:string)  [unwired: 13 in]
        n284 = call <vilib>:"Add State(s) to Queue__JKI_lib_State_Machine.vi"("State(s) in Front (\"\")"=w547, "State(s) in (\"\")"=w588) -> ("States Out"=w587:string)  [unwired: 13 in]
      }
      frame "Macro: Close" {
        w595 = FALSE ("打开串口")
        n285 = Unbundle By Name(w597) -> ("温控情况.打开串口"=w592:bool, "开关信息.开关 1"=w589:bool, "开关信息.开关 2"=w590:bool, "设备信息.双通道设备？"=w593:bool, "基本信息.USB Port"=w594:refnum<visa-resource-name>)
        n286 = And(x=w590, y=w593) -> (x .and. y?=w591:bool)
        n287 = case shown="真" w592 {
          tunnel: w594 -> [_ w606]
          tunnel: w591 -> [_ w614]
          tunnel: w599 -> [w602 w603]
          tunnel: [w602 w609] -> w598
          tunnel: w589 -> [_ w608]
          frame False {
          }
          frame True {
            n288 = property class="Instr"(reference=w606, error in=w603, "General Settings:Timeout Value"=u32 2000) -> (reference out=w605:refnum<visa-resource-name>, error out=w604:errorcluster)
            n289 = case shown="真" w608 {
              tunnel: w605 -> [w616 w621]
              tunnel: [w616 w619] -> w613
              tunnel: [w615 w618] -> w610
              tunnel: w604 -> [w615 w617]
              frame False {
              }
              frame True {
                n290 = call "串口读写 - WK.vi"("错误输入（无错误）"=w617, "写入设备"="TC1:TCSW=0\r" ("写入缓冲区"), "VISA输入"=w621) -> ("错误输出"=w618:errorcluster, "VISA输出"=w619:refnum<visa-resource-name>)  [unwired: 5 in, 2 out]
              }
            }
            n291 = case shown="真" w614 {
              tunnel: w613 -> [w623 w627]
              tunnel: w610 -> [w622 w626]
              tunnel: [w622 w625] -> w612
              tunnel: [w623 w624] -> w611
              frame False {
              }
              frame True {
                n292 = call "串口读写 - WK.vi"("错误输入（无错误）"=w626, "写入设备"="TC2:TCSW=0\r" ("写入缓冲区"), "VISA输入"=w627) -> ("错误输出"=w625:errorcluster, "VISA输出"=w624:refnum<visa-resource-name>)  [unwired: 5 in, 2 out]
              }
            }
            n293 = VISA Close(VISA resource name=w611, error in (no error)=w612) -> (error out=w609:errorcluster)
          }
        }
        n294 = local write "温控开关 1"(w595) -> ()
        n295 = local write "温控开关 2"(w595) -> ()
        n296 = local write "打开串口"(w595) -> ()
        n297 = Bundle By Name(cluster=w597, "温控情况.打开串口"=w595, "开关信息.开关 1"=w595, "开关信息.开关 2"=w595, "开关信息.温控是否打开"=w595) -> (w596:T16)
        n298 = call <vilib>:"Add State(s) to Queue__JKI_lib_State_Machine.vi"("State(s) in (\"\")"=w601) -> ("States Out"=w600:string)  [unwired: 14 in]
      }
      frame "Macro: Stop" {
        n299 = call-poly <userlib>:"Build Message with Arguments++.vi"("States With Replace Token"="//Send Message to Other CSM Modules\nAPI: Stop -@ Acquisition - <1>\nAPI: Stop -@ Logging - <1>\n\nMacro: Close", "<1>"=w632) -> ("States"=w629:string)  [unwired: 13 in]
        n300 = call <vilib>:"Add State(s) to Queue__jki_lib_state_machine.vi"("State(s) in Front (\"\")"=w629, "State(s) in (\"\")"=w630) -> ("States Out"=w631:string)  [unwired: 13 in]
      }
      frame "Macro: Exit" {
        w639 = "//Permanent unregistrations\nAcquired Data@Acquisition - <1> >> Data: Update Indicators -><unregister>\nAcquired Data@Acquisition - <1> >> API: Log@Logging - <1> -><unregister>\n\n//Permanent unregistrations\nError Occurred@Acquisition - <1> >> Error Handler -><unregister>\nError Occurred@Logging - <1> >> Error Handler -><unregister>\n\n\n//Exit\nMacro: Exit-@Logging - <1>\nMacro: Exit-@Acquisition - <1>\n\nMacro: Close\n\nData: Cleanup\nExit"  # //Permanent unregistrations Acquired Data@Acquisition - <1> >> Data: Update Indicators -><unregister> Acquired Data@Acquisition - <1> >> API: Log@Logging - <1> -><unregister>  //Permanent unregistrations Error Occurred@Acquisition - <1> >> Error Handler -><unregister> Error Occurred@Logging - <1> >> Error Handler -><unregister>   //Exit Macro: Exit-@Logging - <1> Macro: Exit-@Acquisition - <1>  Macro: Close  Data: Cleanup Exit
        # "#CSM \"Macro: Exit\"\nExit Macro (This is called once, when the VI exits)"
        n301 = property on="温控循环功能开启" class="Bool (严格)"("Val(Sgnl)"=FALSE ("值(信号)")) -> ()  [unwired: 2 in, 2 out]
        n302 = call-poly <userlib>:"Build Message with Arguments++.vi"("States With Replace Token"=w639, "<1>"=w640) -> ("States"=w636:string)  [unwired: 13 in]
        n303 = call <vilib>:"Add State(s) to Queue__JKI_lib_State_Machine.vi"("State(s) in Front (\"\")"=w636, "State(s) in (\"\")"=w642) -> ("States Out"=w641:string)  [unwired: 13 in]
      }
      frame "---------- Action ----------" {
        # "#CSM \"Category Seperator\"\nDo not put any code in this frame."
        n304 = call <vilib>:"Add State(s) to Queue__JKI_lib_State_Machine.vi"("State(s) in (\"\")"=w645) -> ("States Out"=w644:string)  [unwired: 14 in]
      }
      frame "Action: Power Output 1" {
        # "#CSM \"Internal State\"\nThis category is used for holding internal states"
        n305 = call "Convert API String Arguments to Data.vim"("Reference Type"=FALSE, "API String"=w655) -> ("Data"=w649:bool)  [unwired: 6 in, 1 out]
        n306 = Unbundle By Name(w652) -> ("基本信息.USB Port"=w661:refnum<visa-resource-name>)
        n307 = Boolean To (0,1)(Boolean=w649) -> (0, 1=w657:i16)
        n308 = Number To Decimal String(number=w657) -> (decimal integer string=w653:string)  [unwired: 1 in]
        n309 = local write "温控开关 1"(w649) -> ()
        n310 = Concatenate Strings("TC1:TCSW=" ("写入缓冲区"), w653, "\r" ("写入缓冲区")) -> (w658:string)
        n311 = call "串口读写 - WK.vi"("错误输入（无错误）"=w656, "写入设备"=w658, "VISA输入"=w661) -> ("错误输出"=w650:errorcluster)  [unwired: 5 in, 3 out]
        n312 = Bundle By Name(cluster=w652, "输出参数.输出状态 1.功率输出"=w657, "开关信息.开关 1"=w649) -> (w651:T16)
        n313 = call "Convert Data To API String Arguments.vim"("Data"=w649) -> ("API String"=w648:string)  [unwired: 7 in, 1 out]
        n314 = call <vilib>:"Build State String with Arguments__JKI_lib_State_Machine.vi"("Arguments (\"\")"=w648, "State"="Acq: ONOFF1") -> ("State with Arguments"=w646:string)  [unwired: 4 in]
        n315 = call <vilib>:"Add State(s) to Queue__JKI_lib_State_Machine.vi"("State(s) in Front (\"\")"=w646, "State(s) in (\"\")"=w663) -> ("States Out"=w662:string)  [unwired: 13 in]
      }
      frame "Action: Power Output 2" {
        # "#CSM \"Internal State\"\nThis category is used for holding internal states"
        n316 = Unbundle By Name(w670) -> ("基本信息.USB Port"=w679:refnum<visa-resource-name>)
        n317 = call "Convert API String Arguments to Data.vim"("Reference Type"=FALSE, "API String"=w673) -> ("Data"=w665:bool)  [unwired: 6 in, 1 out]
        n318 = Boolean To (0,1)(Boolean=w665) -> (0, 1=w675:i16)
        n319 = local write "温控开关 2"(w665) -> ()
        n320 = Number To Decimal String(number=w675) -> (decimal integer string=w671:string)  [unwired: 1 in]
        n321 = Concatenate Strings("TC2:TCSW=" ("写入缓冲区"), w671, "\r" ("写入缓冲区")) -> (w676:string)
        n322 = call "串口读写 - WK.vi"("错误输入（无错误）"=w674, "写入设备"=w676, "VISA输入"=w679) -> ("错误输出"=w668:errorcluster)  [unwired: 5 in, 3 out]
        n323 = Bundle By Name(cluster=w670, "输出参数.输出状态 2.功率输出"=w675, "开关信息.开关 2"=w665) -> (w669:T16)
        n324 = call "Convert Data To API String Arguments.vim"("Data"=w665) -> ("API String"=w667:string)  [unwired: 7 in, 1 out]
        n325 = call <vilib>:"Build State String with Arguments__JKI_lib_State_Machine.vi"("Arguments (\"\")"=w667, "State"="Acq: ONOFF2") -> ("State with Arguments"=w664:string)  [unwired: 4 in]
        n326 = call <vilib>:"Add State(s) to Queue__JKI_lib_State_Machine.vi"("State(s) in Front (\"\")"=w664, "State(s) in (\"\")"=w681) -> ("States Out"=w680:string)  [unwired: 13 in]
      }
      frame "Action: Change Temp 1" {
        # "\"API: Control Temp 1\""
        n327 = Unbundle By Name(w698) -> ("基本信息.USB Port"=w704:refnum<visa-resource-name>)
        n328 = local read "过温 1"() -> (w693:T6)
        n329 = call "Convert API String Arguments to Data.vim"("Reference Type"=0.0, "API String"=w685) -> ("Data"=w691:dbl)  [unwired: 6 in, 1 out]
        n330 = Unbundle By Name(w693) -> ("最高设定温度"=w689:dbl, "最低设定温度"=w688:dbl)
        n331 = In Range and Coerce(upper limit=w689, x=w691, lower limit=w688) -> (coerced(x)=w690:dbl)  [unwired: 1 out]
        n332 = Add(x=w690, y=0.0) -> (x+y=w684:dbl)
        n333 = Number To Fractional String(number=w684, precision (6)=i16 2 ("精度(6)")) -> (F-format string=w700:string)  [unwired: 2 in]
        n334 = Concatenate Strings("TC1:TCADJUSTTEMP=" ("写入缓冲区"), w700, "\r" ("写入缓冲区")) -> (w701:string)
        n335 = call "串口读写 - WK.vi"("错误输入（无错误）"=w694, "写入设备"=w701, "VISA输入"=w704) -> ("错误输出"=w696:errorcluster)  [unwired: 5 in, 3 out]
        n336 = local write "温控温度 1"(w684) -> ()
        n337 = Bundle By Name(cluster=w698, "温控情况.温控温度 1"=w684) -> (w697:T16)
        n338 = call "Convert Data To API String Arguments.vim"("Data"=w684) -> ("API String"=w683:string)  [unwired: 7 in, 1 out]
        n339 = call-poly <userlib>:"Build Message with Arguments++.vi"("States With Replace Token"="//Send Message to Other CSM Modules\nAPI: Control Temp 1 >> <param> -@ Acquisition - <1>", "<param>"=w683, "<1>"=w682) -> ("States"=w686:string)  [unwired: 12 in]
        n340 = call <vilib>:"Add State(s) to Queue__JKI_lib_State_Machine.vi"("State(s) in Front (\"\")"=w686, "State(s) in (\"\")"=w706) -> ("States Out"=w705:string)  [unwired: 13 in]
      }
      frame "Action: Change Temp 2" {
        # "#CSM \"Internal State\"\nThis category is used for holding internal states"
        n341 = Unbundle By Name(w715) -> ("设备信息.双通道设备？"=w709:bool, "基本信息.USB Port"=w716:refnum<visa-resource-name>)
        n342 = case shown="真" w709 {
          tunnel: w716 -> [_ w742]
          tunnel: [w721 w736] -> w713
          tunnel: w712 -> [_ w735]
          tunnel: w711 -> [w721 w733]
          tunnel: [25.0 ("Data") w724] -> w710
          tunnel: ["" ("States") w723] -> w708
          tunnel: w707 -> [_ w722]
          frame False {
          }
          frame True {
            n343 = local read "过温 2"() -> (w729:T6)
            n344 = Unbundle By Name(w729) -> ("最高设定温度"=w730:dbl, "最低设定温度"=w731:dbl)
            n345 = call "Convert API String Arguments to Data.vim"("Reference Type"=0.0, "API String"=w735) -> ("Data"=w727:dbl)  [unwired: 6 in, 1 out]
            n346 = In Range and Coerce(upper limit=w730, x=w727, lower limit=w731) -> (coerced(x)=w732:dbl)  [unwired: 1 out]
            n347 = Add(x=w732, y=0.0) -> (x+y=w724:dbl)
            n348 = Number To Fractional String(number=w724, precision (6)=i16 2 ("精度(6)")) -> (F-format string=w738:string)  [unwired: 2 in]
            n349 = Concatenate Strings("TC2:TCADJUSTTEMP=" ("写入缓冲区"), w738, "\r" ("写入缓冲区")) -> (w739:string)
            n350 = call "串口读写 - WK.vi"("错误输入（无错误）"=w733, "写入设备"=w739, "VISA输入"=w742) -> ("错误输出"=w736:errorcluster)  [unwired: 5 in, 3 out]
            n351 = call "Convert Data To API String Arguments.vim"("Data"=w724) -> ("API String"=w726:string)  [unwired: 7 in, 1 out]
            n352 = call-poly <userlib>:"Build Message with Arguments++.vi"("States With Replace Token"="//Send Message to Other CSM Modules\nAPI: Control Temp 1 >> <param> -@ Acquisition - <1>", "<param>"=w726, "<1>"=w722) -> ("States"=w723:string)  [unwired: 12 in]
          }
        }
        n353 = local write "温控温度 2"(w710) -> ()
        n354 = Bundle By Name(cluster=w715, "温控情况.温控温度 2"=w710) -> (w714:T16)
        n355 = call <vilib>:"Add State(s) to Queue__JKI_lib_State_Machine.vi"("State(s) in Front (\"\")"=w708, "State(s) in (\"\")"=w718) -> ("States Out"=w717:string)  [unwired: 13 in]
      }
      frame "Action: Power Switch 1" {
        # "#CSM \"Internal State\"\nThis category is used for holding internal states"
        n356 = call "Convert API String Arguments to Data.vim"("Reference Type"=FALSE, "API String"=w750) -> ("Data"=w744:bool)  [unwired: 6 in, 1 out]
        n357 = Unbundle By Name(w747) -> ("基本信息.USB Port"=w755:refnum<visa-resource-name>)
        n358 = Boolean To (0,1)(Boolean=w744) -> (0, 1=w743:i16)
        n359 = Number To Decimal String(number=w743) -> (decimal integer string=w748:string)  [unwired: 1 in]
        n360 = local write "温控开关 1"(w744) -> ()
        n361 = Concatenate Strings("TC1:TCSW=" ("写入缓冲区"), w748, "\r" ("写入缓冲区")) -> (w752:string)
        n362 = call "串口读写 - WK.vi"("错误输入（无错误）"=w751, "写入设备"=w752, "VISA输入"=w755) -> ("错误输出"=w745:errorcluster)  [unwired: 5 in, 3 out]
        n363 = Bundle By Name(cluster=w747, "输出参数.输出状态 1.功率输出"=w743, "开关信息.开关 1"=w744) -> (w746:T16)
        n364 = property on="过压/过流 1" class="Clust (严格)"("DisabledEnum"=w743) -> ()  [unwired: 2 in, 2 out]
        n365 = property on="输出设置 1" class="Clust (严格)"("DisabledEnum"=w743) -> ()  [unwired: 2 in, 2 out]
        n366 = call <vilib>:"Add State(s) to Queue__JKI_lib_State_Machine.vi"("State(s) in (\"\")"=w757) -> ("States Out"=w756:string)  [unwired: 14 in]
      }
      frame "Action: Power Switch 2" {
        # "#CSM \"Internal State\"\nThis category is used for holding internal states"
        n367 = Unbundle By Name(w762) -> ("基本信息.USB Port"=w770:refnum<visa-resource-name>)
        n368 = call "Convert API String Arguments to Data.vim"("Reference Type"=FALSE, "API String"=w765) -> ("Data"=w759:bool)  [unwired: 6 in, 1 out]
        n369 = Boolean To (0,1)(Boolean=w759) -> (0, 1=w758:i16)
        n370 = local write "温控开关 2"(w759) -> ()
        n371 = Number To Decimal String(number=w758) -> (decimal integer string=w763:string)  [unwired: 1 in]
        n372 = Concatenate Strings("TC2:TCSW=" ("写入缓冲区"), w763, "\r" ("写入缓冲区")) -> (w767:string)
        n373 = call "串口读写 - WK.vi"("错误输入（无错误）"=w766, "写入设备"=w767, "VISA输入"=w770) -> ("错误输出"=w760:errorcluster)  [unwired: 5 in, 3 out]
        n374 = Bundle By Name(cluster=w762, "输出参数.输出状态 2.功率输出"=w758, "开关信息.开关 2"=w759) -> (w761:T16)
        n375 = property on="过压/过流 2" class="Clust (严格)"("DisabledEnum"=w758) -> ()  [unwired: 2 in, 2 out]
        n376 = property on="输出设置 2" class="Clust (严格)"("DisabledEnum"=w758) -> ()  [unwired: 2 in, 2 out]
        n377 = call <vilib>:"Add State(s) to Queue__JKI_lib_State_Machine.vi"("State(s) in (\"\")"=w772) -> ("States Out"=w771:string)  [unwired: 14 in]
      }
      frame "Action: Output Set 1" {
        w778 = "/" ("字符串")
        n378 = call "Convert API String Arguments to Data.vim"("Reference Type"=w778, "error in (no error)"=w774, "API String"=w780) -> ("error out"=w777:errorcluster, "Data"=w779:string)  [unwired: 5 in]
        n379 = Unbundle By Name(w776) -> ("基本信息.USB Port"=w791:refnum<visa-resource-name>)
        n380 = Match Pattern(string=w779, regular expression=w778) -> (before substring=w787:string, after substring=w785:string)  [unwired: 1 in, 2 out]
        n381 = Fract/Exp String To Number(string=w785) -> (number=w784:dbl)  [unwired: 3 in, 1 out]
        n382 = case shown="\"1\"" w787 {
          tunnel: ["TC1:TCMODE" ("写入缓冲区") "TC1:TCMAXV" ("写入缓冲区")] -> w786
          tunnel: w776 -> [w794 w798]
          tunnel: [w793 w797] -> w775
          tunnel: w784 -> [w792 w796]
          frame "1" {
            n383 = Bundle By Name(cluster=w794, "输出参数.输出设置 1.输出模式"=w792) -> (w793:T16)
          }
          frame "2", Default {
            n384 = Bundle By Name(cluster=w798, "输出参数.输出设置 1.最大输出电压"=w796) -> (w797:T16)
          }
        }
        n385 = Concatenate Strings(w786, "=" ("写入缓冲区"), w785, "\r" ("写入缓冲区")) -> (w788:string)
        n386 = call "串口读写 - WK.vi"("错误输入（无错误）"=w777, "是否保存?(F)"=FALSE ("是否保存？"), "写入设备"=w788, "VISA输入"=w791) -> ("错误输出"=w773:errorcluster)  [unwired: 4 in, 3 out]
        n387 = call <vilib>:"Add State(s) to Queue__JKI_lib_State_Machine.vi"("State(s) in (\"\")"=w781) -> ("States Out"=w782:string)  [unwired: 14 in]
      }
      frame "Action: Output Set 2" {
        w805 = "/" ("字符串")
        n388 = call "Convert API String Arguments to Data.vim"("Reference Type"=w805, "error in (no error)"=w801, "API String"=w807) -> ("error out"=w804:errorcluster, "Data"=w806:string)  [unwired: 5 in]
        n389 = Unbundle By Name(w803) -> ("基本信息.USB Port"=w818:refnum<visa-resource-name>)
        n390 = Match Pattern(string=w806, regular expression=w805) -> (before substring=w814:string, after substring=w812:string)  [unwired: 1 in, 2 out]
        n391 = Fract/Exp String To Number(string=w812) -> (number=w811:dbl)  [unwired: 3 in, 1 out]
        n392 = case shown="\"2\", 默认" w814 {
          tunnel: ["TC2:TCMODE" ("写入缓冲区") "TC2:TCMAXV" ("写入缓冲区")] -> w813
          tunnel: w803 -> [w821 w825]
          tunnel: [w820 w824] -> w802
          tunnel: w811 -> [w819 w823]
          frame "1" {
            n393 = Bundle By Name(cluster=w821, "输出参数.输出设置 2.输出模式"=w819) -> (w820:T16)
          }
          frame "2", Default {
            n394 = Bundle By Name(cluster=w825, "输出参数.输出设置 2.最大输出电压"=w823) -> (w824:T16)
          }
        }
        n395 = Concatenate Strings(w813, "=" ("写入缓冲区"), w812, "\r" ("写入缓冲区")) -> (w815:string)
        n396 = call "串口读写 - WK.vi"("错误输入（无错误）"=w804, "是否保存?(F)"=FALSE ("是否保存？"), "写入设备"=w815, "VISA输入"=w818) -> ("错误输出"=w800:errorcluster)  [unwired: 4 in, 3 out]
        n397 = call <vilib>:"Add State(s) to Queue__JKI_lib_State_Machine.vi"("State(s) in (\"\")"=w808) -> ("States Out"=w809:string)  [unwired: 14 in]
      }
      frame "Action: PID Set 1" {
        w835 = "/" ("字符串")
        n398 = call "Convert API String Arguments to Data.vim"("Reference Type"=w835, "error in (no error)"=w833, "API String"=w837) -> ("error out"=w834:errorcluster, "Data"=w836:string)  [unwired: 5 in]
        n399 = Unbundle By Name(w831) -> ("基本信息.USB Port"=w845:refnum<visa-resource-name>)
        n400 = Match Pattern(string=w836, regular expression=w835) -> (before substring=w829:string, after substring=w841:string)  [unwired: 1 in, 2 out]
        n401 = Fract/Exp String To Number(string=w841) -> (number=w830:dbl)  [unwired: 3 in, 1 out]
        n402 = case shown="\"32\"" w829 {
          tunnel: ["" ("写入缓冲区") "TC1:TCPIDTYPE" ("写入缓冲区") "TC1:TCP" ("写入缓冲区") "TC1:TCTI" ("写入缓冲区") "TC1:TCTD" ("写入缓冲区") "TC1:TCCTRLINTERVAL" ("写入缓冲区") "TC1:TCPIDCAL" ("写入缓冲区")] -> w828
          tunnel: w831 -> [w847 w850 w854 w858 w862 w866 w870]
          tunnel: [w847 w849 w853 w857 w861 w865 w869] -> w827
          tunnel: w830 -> [_ w848 w852 w856 w860 w864 w868]
          frame "0", Default {
          }
          frame "1" {
            n403 = Bundle By Name(cluster=w850, "输出参数.PID 1.PID类型"=w848) -> (w849:T16)
          }
          frame "2" {
            n404 = Bundle By Name(cluster=w854, "输出参数.PID 1.P"=w852) -> (w853:T16)
          }
          frame "4" {
            n405 = Bundle By Name(cluster=w858, "输出参数.PID 1.I"=w856) -> (w857:T16)
          }
          frame "8" {
            n406 = Bundle By Name(cluster=w862, "输出参数.PID 1.D"=w860) -> (w861:T16)
          }
          frame "16" {
            n407 = Bundle By Name(cluster=w866, "输出参数.PID 1.PID控制间隔"=w864) -> (w865:T16)
          }
          frame "32" {
            n408 = Bundle By Name(cluster=w870, "输出参数.PID 1.PID计算方法"=w868) -> (w869:T16)
          }
        }
        n409 = Concatenate Strings(w828, "=" ("写入缓冲区"), w841, "\r" ("写入缓冲区")) -> (w842:string)
        n410 = call "串口读写 - WK.vi"("错误输入（无错误）"=w834, "是否保存?(F)"=FALSE ("是否保存？"), "写入设备"=w842, "VISA输入"=w845) -> ("错误输出"=w832:errorcluster)  [unwired: 4 in, 3 out]
        n411 = call <vilib>:"Add State(s) to Queue__JKI_lib_State_Machine.vi"("State(s) in (\"\")"=w838) -> ("States Out"=w839:string)  [unwired: 14 in]
      }
      frame "Action: PID Set 2" {
        w880 = "/" ("字符串")
        n412 = call "Convert API String Arguments to Data.vim"("Reference Type"=w880, "error in (no error)"=w878, "API String"=w882) -> ("error out"=w879:errorcluster, "Data"=w881:string)  [unwired: 5 in]
        n413 = Unbundle By Name(w874) -> ("基本信息.USB Port"=w890:refnum<visa-resource-name>)
        n414 = Match Pattern(string=w881, regular expression=w880) -> (before substring=w875:string, after substring=w886:string)  [unwired: 1 in, 2 out]
        n415 = Fract/Exp String To Number(string=w886) -> (number=w876:dbl)  [unwired: 3 in, 1 out]
        n416 = case shown="\"0\", 默认" w875 {
          tunnel: ["" ("写入缓冲区") "TC2:TCPIDTYPE" ("写入缓冲区") "TC2:TCP" ("写入缓冲区") "TC2:TCTI" ("写入缓冲区") "TC2:TCTD" ("写入缓冲区") "TC2:TCCTRLINTERVAL" ("写入缓冲区") "TC2:TCPIDCAL" ("写入缓冲区")] -> w872
          tunnel: w874 -> [w892 w895 w899 w903 w907 w911 w915]
          tunnel: [w892 w894 w898 w902 w906 w910 w914] -> w873
          tunnel: w876 -> [_ w893 w897 w901 w905 w909 w913]
          frame "0", Default {
          }
          frame "1" {
            n417 = Bundle By Name(cluster=w895, "输出参数.PID 2.PID类型"=w893) -> (w894:T16)
          }
          frame "2" {
            n418 = Bundle By Name(cluster=w899, "输出参数.PID 2.P"=w897) -> (w898:T16)
          }
          frame "4" {
            n419 = Bundle By Name(cluster=w903, "输出参数.PID 2.I"=w901) -> (w902:T16)
          }
          frame "8" {
            n420 = Bundle By Name(cluster=w907, "输出参数.PID 2.D"=w905) -> (w906:T16)
          }
          frame "16" {
            n421 = Bundle By Name(cluster=w911, "输出参数.PID 2.PID控制间隔"=w909) -> (w910:T16)
          }
          frame "32" {
            n422 = Bundle By Name(cluster=w915, "输出参数.PID 2.PID计算方法"=w913) -> (w914:T16)
          }
        }
        n423 = Concatenate Strings(w872, "=" ("写入缓冲区"), w886, "\r" ("写入缓冲区")) -> (w887:string)
        n424 = call "串口读写 - WK.vi"("错误输入（无错误）"=w879, "是否保存?(F)"=FALSE ("是否保存？"), "写入设备"=w887, "VISA输入"=w890) -> ("错误输出"=w877:errorcluster)  [unwired: 4 in, 3 out]
        n425 = call <vilib>:"Add State(s) to Queue__JKI_lib_State_Machine.vi"("State(s) in (\"\")"=w883) -> ("States Out"=w884:string)  [unwired: 14 in]
      }
      frame "Action: OTP Set 1" {
        w925 = "/" ("字符串")
        n426 = call "Convert API String Arguments to Data.vim"("Reference Type"=w925, "error in (no error)"=w923, "API String"=w927) -> ("error out"=w924:errorcluster, "Data"=w926:string)  [unwired: 5 in]
        n427 = Unbundle By Name(w920) -> ("基本信息.USB Port"=w935:refnum<visa-resource-name>)
        n428 = Match Pattern(string=w926, regular expression=w925) -> (before substring=w921:string, after substring=w931:string)  [unwired: 1 in, 2 out]
        n429 = Fract/Exp String To Number(string=w931) -> (number=w919:dbl)  [unwired: 3 in, 1 out]
        n430 = case shown="\"1\"" w921 {
          tunnel: ["" ("写入缓冲区") "TC1:TCOTPE" ("写入缓冲区") "TC1:TCOTPLT" ("写入缓冲区") "TC1:TCOTPHT" ("写入缓冲区") "TC1:TCMINSETTEMP" ("写入缓冲区") "TC1:TCMAXSETTEMP" ("写入缓冲区") "TC1:TCRAMPSPEED" ("写入缓冲区")] -> w917
          tunnel: w920 -> [w937 w941 w945 w949 w953 w957 w961]
          tunnel: [w937 w940 w944 w948 w952 w956 w960] -> w918
          tunnel: w919 -> [_ w939 w943 w947 w951 w955 w959]
          frame "0", Default {
          }
          frame "1" {
            n431 = Not Equal To 0?(x=w939) -> (x != 0?=w938:bool)
            n432 = Bundle By Name(cluster=w941, "保护.过温 1.过温保护开关"=w938) -> (w940:T16)
          }
          frame "2" {
            n433 = Bundle By Name(cluster=w945, "保护.过温 1.过温保护低阈值"=w943) -> (w944:T16)
          }
          frame "4" {
            n434 = Bundle By Name(cluster=w949, "保护.过温 1.过温保护高阈值"=w947) -> (w948:T16)
          }
          frame "8" {
            n435 = Bundle By Name(cluster=w953, "保护.过温 1.最低设定温度"=w951) -> (w952:T16)
          }
          frame "16" {
            n436 = Bundle By Name(cluster=w957, "保护.过温 1.最高设定温度"=w955) -> (w956:T16)
          }
          frame "32" {
            n437 = Bundle By Name(cluster=w961, "保护.过温 1.温度限速"=w959) -> (w960:T16)
          }
        }
        n438 = Concatenate Strings(w917, "=" ("写入缓冲区"), w931, "\r" ("写入缓冲区")) -> (w932:string)
        n439 = call "串口读写 - WK.vi"("错误输入（无错误）"=w924, "是否保存?(F)"=FALSE ("是否保存？"), "写入设备"=w932, "VISA输入"=w935) -> ("错误输出"=w922:errorcluster)  [unwired: 4 in, 3 out]
        n440 = call <vilib>:"Add State(s) to Queue__JKI_lib_State_Machine.vi"("State(s) in (\"\")"=w928) -> ("States Out"=w929:string)  [unwired: 14 in]
      }
      frame "Action: OTP Set 2" {
        w971 = "/" ("字符串")
        n441 = call "Convert API String Arguments to Data.vim"("Reference Type"=w971, "error in (no error)"=w969, "API String"=w973) -> ("error out"=w970:errorcluster, "Data"=w972:string)  [unwired: 5 in]
        n442 = Unbundle By Name(w967) -> ("基本信息.USB Port"=w981:refnum<visa-resource-name>)
        n443 = Match Pattern(string=w972, regular expression=w971) -> (before substring=w966:string, after substring=w977:string)  [unwired: 1 in, 2 out]
        n444 = Fract/Exp String To Number(string=w977) -> (number=w965:dbl)  [unwired: 3 in, 1 out]
        n445 = case shown="\"0\", 默认" w966 {
          tunnel: ["" ("写入缓冲区") "TC2:TCOTPE" ("写入缓冲区") "TC2:TCOTPLT" ("写入缓冲区") "TC2:TCOTPHT" ("写入缓冲区") "TC2:TCMINSETTEMP" ("写入缓冲区") "TC2:TCMAXSETTEMP" ("写入缓冲区") "TC2:TCRAMPSPEED" ("写入缓冲区")] -> w964
          tunnel: w967 -> [w983 w987 w991 w995 w999 w1003 w1007]
          tunnel: [w983 w986 w990 w994 w998 w1002 w1006] -> w963
          tunnel: w965 -> [_ w985 w989 w993 w997 w1001 w1005]
          frame "0", Default {
          }
          frame "1" {
            n446 = Not Equal To 0?(x=w985) -> (x != 0?=w984:bool)
            n447 = Bundle By Name(cluster=w987, "保护.过温 2.过温保护开关"=w984) -> (w986:T16)
          }
          frame "2" {
            n448 = Bundle By Name(cluster=w991, "保护.过温 2.过温保护低阈值"=w989) -> (w990:T16)
          }
          frame "4" {
            n449 = Bundle By Name(cluster=w995, "保护.过温 2.过温保护高阈值"=w993) -> (w994:T16)
          }
          frame "8" {
            n450 = Bundle By Name(cluster=w999, "保护.过温 2.最低设定温度"=w997) -> (w998:T16)
          }
          frame "16" {
            n451 = Bundle By Name(cluster=w1003, "保护.过温 2.最高设定温度"=w1001) -> (w1002:T16)
          }
          frame "32" {
            n452 = Bundle By Name(cluster=w1007, "保护.过温 2.温度限速"=w1005) -> (w1006:T16)
          }
        }
        n453 = Concatenate Strings(w964, "=" ("写入缓冲区"), w977, "\r" ("写入缓冲区")) -> (w978:string)
        n454 = call "串口读写 - WK.vi"("错误输入（无错误）"=w970, "是否保存?(F)"=FALSE ("是否保存？"), "写入设备"=w978, "VISA输入"=w981) -> ("错误输出"=w968:errorcluster)  [unwired: 4 in, 3 out]
        n455 = call <vilib>:"Add State(s) to Queue__JKI_lib_State_Machine.vi"("State(s) in (\"\")"=w974) -> ("States Out"=w975:string)  [unwired: 14 in]
      }
      frame "Action: OVP Set 1" {
        w1017 = "/" ("字符串")
        n456 = call "Convert API String Arguments to Data.vim"("Reference Type"=w1017, "error in (no error)"=w1015, "API String"=w1019) -> ("error out"=w1016:errorcluster, "Data"=w1018:string)  [unwired: 5 in]
        n457 = Unbundle By Name(w1011) -> ("基本信息.USB Port"=w1027:refnum<visa-resource-name>)
        n458 = Match Pattern(string=w1018, regular expression=w1017) -> (before substring=w1010:string, after substring=w1023:string)  [unwired: 1 in, 2 out]
        n459 = Fract/Exp String To Number(string=w1023) -> (number=w1009:dbl)  [unwired: 3 in, 1 out]
        n460 = case shown="\"2\"" w1010 {
          tunnel: ["" ("写入缓冲区") "TC1:TCADJUSTOVPV" ("写入缓冲区") "TC1:TCADJUSTOCPC" ("写入缓冲区")] -> w1013
          tunnel: w1011 -> [w1029 w1032 w1036]
          tunnel: [w1029 w1031 w1035] -> w1012
          tunnel: w1009 -> [_ w1030 w1034]
          frame "0", Default {
          }
          frame "1" {
            n461 = Bundle By Name(cluster=w1032, "保护.过压/过流 1.过压保护阈值"=w1030) -> (w1031:T16)
          }
          frame "2" {
            n462 = Bundle By Name(cluster=w1036, "保护.过压/过流 1.过流保护阈值"=w1034) -> (w1035:T16)
          }
        }
        n463 = Concatenate Strings(w1013, "=" ("写入缓冲区"), w1023, "\r" ("写入缓冲区")) -> (w1024:string)
        n464 = call "串口读写 - WK.vi"("错误输入（无错误）"=w1016, "是否保存?(F)"=FALSE ("是否保存？"), "写入设备"=w1024, "VISA输入"=w1027) -> ("错误输出"=w1014:errorcluster)  [unwired: 4 in, 3 out]
        n465 = call <vilib>:"Add State(s) to Queue__JKI_lib_State_Machine.vi"("State(s) in (\"\")"=w1020) -> ("States Out"=w1021:string)  [unwired: 14 in]
      }
      frame "Action: OVP Set 2" {
        w1046 = "/" ("字符串")
        n466 = call "Convert API String Arguments to Data.vim"("Reference Type"=w1046, "error in (no error)"=w1044, "API String"=w1048) -> ("error out"=w1045:errorcluster, "Data"=w1047:string)  [unwired: 5 in]
        n467 = Unbundle By Name(w1040) -> ("基本信息.USB Port"=w1056:refnum<visa-resource-name>)
        n468 = Match Pattern(string=w1047, regular expression=w1046) -> (before substring=w1039:string, after substring=w1052:string)  [unwired: 1 in, 2 out]
        n469 = Fract/Exp String To Number(string=w1052) -> (number=w1038:dbl)  [unwired: 3 in, 1 out]
        n470 = case shown="\"1\"" w1039 {
          tunnel: ["" ("写入缓冲区") "TC2:TCADJUSTOVPV" ("写入缓冲区") "TC2:TCADJUSTOCPC" ("写入缓冲区")] -> w1042
          tunnel: w1040 -> [w1058 w1061 w1065]
          tunnel: [w1058 w1060 w1064] -> w1041
          tunnel: w1038 -> [_ w1059 w1063]
          frame "0", Default {
          }
          frame "1" {
            n471 = Bundle By Name(cluster=w1061, "保护.过压/过流 2.过压保护阈值"=w1059) -> (w1060:T16)
          }
          frame "2" {
            n472 = Bundle By Name(cluster=w1065, "保护.过压/过流 2.过流保护阈值"=w1063) -> (w1064:T16)
          }
        }
        n473 = Concatenate Strings(w1042, "=" ("写入缓冲区"), w1052, "\r" ("写入缓冲区")) -> (w1053:string)
        n474 = call "串口读写 - WK.vi"("错误输入（无错误）"=w1045, "是否保存?(F)"=FALSE ("是否保存？"), "写入设备"=w1053, "VISA输入"=w1056) -> ("错误输出"=w1043:errorcluster)  [unwired: 4 in, 3 out]
        n475 = call <vilib>:"Add State(s) to Queue__JKI_lib_State_Machine.vi"("State(s) in (\"\")"=w1049) -> ("States Out"=w1050:string)  [unwired: 14 in]
      }
      frame "---------- Acq ----------" {
        # "#CSM \"Category Seperator\"\nDo not put any code in this frame."
      }
      frame "Acq: Fast Mode" {
        n476 = call-poly <userlib>:"Build Message with Arguments++.vi"("States With Replace Token"="API: Fast Mode >> <param> ->| Acquisition - <1>" ("State"), "<param>"=w1073, "<1>"=w1072) -> ("States"=w1069:string)  [unwired: 12 in]
        n477 = call <vilib>:"Add State(s) to Queue__JKI_lib_State_Machine.vi"("State(s) in Front (\"\")"=w1069, "State(s) in (\"\")"=w1070) -> ("States Out"=w1071:string)  [unwired: 13 in]
      }
      frame "Acq: ONOFF1" {
        n478 = call-poly <userlib>:"Build Message with Arguments++.vi"("States With Replace Token"="API: ONOFF1 >> <param> ->| Acquisition - <1>" ("State"), "<param>"=w1081, "<1>"=w1080) -> ("States"=w1077:string)  [unwired: 12 in]
        n479 = call <vilib>:"Add State(s) to Queue__JKI_lib_State_Machine.vi"("State(s) in Front (\"\")"=w1077, "State(s) in (\"\")"=w1078) -> ("States Out"=w1079:string)  [unwired: 13 in]
      }
      frame "Acq: ONOFF2" {
        n480 = call-poly <userlib>:"Build Message with Arguments++.vi"("States With Replace Token"="API: ONOFF2 >> <param> ->| Acquisition - <1>" ("State"), "<param>"=w1089, "<1>"=w1088) -> ("States"=w1085:string)  [unwired: 12 in]
        n481 = call <vilib>:"Add State(s) to Queue__JKI_lib_State_Machine.vi"("State(s) in Front (\"\")"=w1085, "State(s) in (\"\")"=w1086) -> ("States Out"=w1087:string)  [unwired: 13 in]
      }
      frame "Acq: Sample Interval" {
        n482 = call-poly <userlib>:"Build Message with Arguments++.vi"("States With Replace Token"="API: Sample Interval >> <param> ->| Acquisition - <1>" ("State"), "<param>"=w1096, "<1>"=w1101) -> ("States"=w1098:string)  [unwired: 12 in]
        n483 = call "Convert API String Arguments to Data.vim"("Reference Type"=0.0, "API String"=w1096) -> ("Data"=w1095:dbl)  [unwired: 6 in, 1 out]
        n484 = Bundle By Name(cluster=w1097, "基本信息.采集间隔(s)"=w1095) -> (w1093:T16)
        n485 = call <vilib>:"Add State(s) to Queue__JKI_lib_State_Machine.vi"("State(s) in Front (\"\")"=w1098, "State(s) in (\"\")"=w1099) -> ("States Out"=w1100:string)  [unwired: 13 in]
      }
      frame "---------- Repeat ----------" {
        # "#CSM \"Internal State\"\nThis category is used for holding internal states"
        n486 = call <vilib>:"Add State(s) to Queue__JKI_lib_State_Machine.vi"("State(s) in (\"\")"=w1106) -> ("States Out"=w1105:string)  [unwired: 14 in]
      }
      frame "Repeat: Enable" {
        w1108 = T22 [{"控制温度"=25.0, "时长(s)"=60.0, "进度"=1.000390362739563, "温控开关"=FALSE}, {"控制温度"=26.0, "时长(s)"=60.0, "进度"=1.0013926823933919, "温控开关"=TRUE}, {"控制温度"=25.0, "时长(s)"=60.0, "进度"=1.0006222248077392, "温控开关"=FALSE}, {"控制温度"=26.0, "时长(s)"=60.0, "进度"=0.6612281163533529, "温控开关"=TRUE}]  # 循环步骤
        # "注意不是簇，是簇的数组，所以不可以用"
        # "#CSM \"Internal State\"\nThis category is used for holding internal states"
        n487 = call "CSM - Read Configuration Variable.vim"("Section Name (\"\" as Default)"=w1107, "Configuration Prototype (Cluster Prefered)"=w1108) -> ("Configuration"=w1109:T22)  [unwired: 6 in, 1 out]
        n488 = Concatenate Strings("Repeat - " ("Name(\"\" to use uuid)"), w1107) -> (w1114:string)
        n489 = control-ref of="子面板-Repeat"() -> (w1117:refnum<vi>)
        n490 = vi-ref "Repeat.vi"() -> (w1116:refnum<vi>)
        n491 = call "Convert Data To API String Arguments.vim"("Data"=w1109) -> ("API String"=w1110:string)  [unwired: 7 in, 1 out]
        n492 = disable-structure shown="禁用" {
          frame Disabled {
            n493 = call "CSM - Read Cluster Elements From Session.vim"() -> ()  [unwired: 8 in, 2 out]
          }
          frame Enabled {
          }
        }
        n494 = call "打开引用WK.vi"("引用"=w1117, "CSM Name"=w1114, "VI"=w1116) -> ("错误输出"=w1112:errorcluster)  [unwired: 7 in, 1 out]
        n495 = flat-sequence {
          tunnel: [w1125] -> w1113
          tunnel: w1107 -> [w1123]
          tunnel: w1112 -> [_]
          tunnel: w1110 -> [w1120]
          frame #0 {
            w1127 = "Error Occurred@Repeat - <1> >> Error Handler -><register>\nRepeat Changed@Repeat - <1> >> Save Repeat -><register>"  # Error Occurred@Repeat - <1> >> Error Handler -><register> Repeat Changed@Repeat - <1> >> Save Repeat -><register>
            n496 = Wait (ms)(milliseconds to wait=u32 100 ("等待时间（毫秒）")) -> ()  [unwired: 1 out]
            n497 = call <vilib>:"Add State(s) to Queue__JKI_lib_State_Machine.vi"("State(s) in Front (\"\")"=w1127, "State(s) in (\"\")"="API: CSM Name  >> <1> ->| Repeat - <1> ", "State(s) at Back (\"\")"="API: INI Read  >> <param> ->| Repeat - <1> ") -> ("States Out"=w1126:string)  [unwired: 12 in]
            n498 = call-poly <userlib>:"Build Message with Arguments++.vi"("States With Replace Token"=w1126, "<param>"=w1120, "<1>"=w1123) -> ("States"=w1125:string)  [unwired: 12 in]
          }
        }
        n499 = call <vilib>:"Add State(s) to Queue__JKI_lib_State_Machine.vi"("State(s) in Front (\"\")"=w1113, "State(s) in (\"\")"=w1119) -> ("States Out"=w1118:string)  [unwired: 13 in]
      }
      frame "Save Repeat" {
        w1131 = T22 [{"控制温度"=25.0, "时长(s)"=60.0, "进度"=1.000390362739563, "温控开关"=FALSE}, {"控制温度"=26.0, "时长(s)"=60.0, "进度"=1.0013926823933919, "温控开关"=TRUE}, {"控制温度"=25.0, "时长(s)"=60.0, "进度"=1.0006222248077392, "温控开关"=FALSE}, {"控制温度"=26.0, "时长(s)"=60.0, "进度"=0.6612281163533529, "温控开关"=TRUE}]  # 循环步骤
        n500 = call "Convert API String Arguments to Data.vim"("Reference Type"=w1131, "API String"=w1130) -> ("Data"=w1129:T22)  [unwired: 6 in, 1 out]
        n501 = call "CSM - Write Configuration Variable.vim"("Section Name (\"\" as Default)"=w1128, "Configuration"=w1129) -> ()  [unwired: 6 in, 2 out]
        n502 = call <vilib>:"Add State(s) to Queue__jki_lib_state_machine.vi"("State(s) in (\"\")"=w1132) -> ("States Out"=w1133:string)  [unwired: 14 in]
      }
      frame "Repeat: Disable" {
        w1140 = "Error Occurred@Repeat - <1> >> Error Handler -><unregister>\nRepeat Changed@Repeat - <1> >> Save Repeat -><unregister>"  # Error Occurred@Repeat - <1> >> Error Handler -><unregister> Repeat Changed@Repeat - <1> >> Save Repeat -><unregister>
        # "#CSM \"Internal State\"\nThis category is used for holding internal states"
        n503 = call <vilib>:"Add State(s) to Queue__JKI_lib_State_Machine.vi"("State(s) in Front (\"\")"=w1140, "State(s) in (\"\")"="Macro: Exit-@Repeat - <1>", "State(s) at Back (\"\")"="Repeat: Remove" ("State(s) at Back (\"\")")) -> ("States Out"=w1138:string)  [unwired: 12 in]
        n504 = call-poly <userlib>:"Build Message with Arguments++.vi"("States With Replace Token"=w1138, "<1>"=w1141) -> ("States"=w1137:string)  [unwired: 13 in]
        n505 = call <vilib>:"Add State(s) to Queue__JKI_lib_State_Machine.vi"("State(s) in Front (\"\")"=w1137, "State(s) in (\"\")"=w1144) -> ("States Out"=w1143:string)  [unwired: 13 in]
      }
      frame "Repeat: Remove" {
        n506 = control-ref of="子面板-Repeat"() -> (w1147:refnum<vi>)
        n507 = invoke class="SubPnl" method="Remove VI"(reference=w1147) -> (error out=w1145:errorcluster)  [unwired: 2 in, 2 out]
        n508 = vi-ref "Repeat.vi"() -> (w1146:refnum<vi>)
        n509 = call "关闭引用WK.vi"("错误输入（无错误）"=w1145, "引用"=w1146) -> ()  [unwired: 9 in, 1 out]
      }
    }
    n510 = Unbundle By Name(w33) -> ("子程序.子程序？"=w32:bool)
    n511 = call "State Delete -WK1.vi"("Delete?(F)"=w32, "CSM name to delete"=string[] ["Logging"], "State In"=w36) -> ("State Out"=w35:string)  [unwired: 8 in]
  }
  n512 = while {
    shift-right: [w1161] -> _
    shift-left: enum16{"Idle", "Initialize", "Exit"}."Initialize" -> [w1162]
    tunnel: "CSM Name" -> [w1159]
    shift-right: [w1157] -> _
    shift-left: w9 -> [w1158]
    shift-right: [w1155] -> _
    shift-left: -1 -> [w1156]
    shift-right: [w1154] -> _
    shift-left: _ -> [w1153]
    shift-right: [w1152] -> _
    shift-left: _ -> [w1151]
    stop <- w1160 stop-if-true
    n513 = case shown="\"Idle\", 默认" w1162 {
      tunnel: [enum16{"Idle", "Initialize", "Exit"}."Idle" w1180 enum16{"Idle", "Initialize", "Exit"}."Exit"] -> w1161
      tunnel: [_ _ TRUE] -> w1160
      tunnel: w1159 -> [w1166 w1179 _]
      tunnel: w1158 -> [w1169 w1177 w1575]
      tunnel: [w1169 w1178 w1575] -> w1157
      tunnel: w1156 -> [_ w1175 _]
      tunnel: [-1 w1176 _] -> w1155
      tunnel: [w1165 w1173 _] -> w1154
      tunnel: w1153 -> [_ w1174 w1574]
      tunnel: [w1163 w1171 w1572] -> w1152
      tunnel: w1151 -> [_ w1172 w1572]
      frame "Initialize" {
        w1164 = FALSE  # your data
        n514 = call <userlib>:"CSM - Module Exit Event.vi"("Name (\"\" to Use UUID) In"=w1166) -> ("CSM Exit Event"=w1167:refnum<user-event>)  [unwired: 8 in, 2 out]
        n515 = register-events(w1167) -> (reference out=w1165:refnum<event-registration>)  [unwired: 2 in, 1 out]
        n516 = Bundle("your data"=w1164) -> (w1163:cluster{"your data":bool})  [unwired: 1 in]
      }
      frame "Idle", Default {
        n517 = event shown="[8] \"温控温度 1\": 值改变" {
          selector: w1174 -> [_ _ _ _ _ _ _ _ _ _ _ _ _ _ _ _ _ _ _ _ _ _ _ _]
          dyn-events: [_ _ _ _ _ _ _ _ _ _ _ _ _ _ _ _ _ _ _ _ _ _ _ _] -> w1173
          timeout: w1175 -> [_ _ _ _ _ _ _ _ _ _ _ _ _ _ _ _ _ _ _ _ _ _ _ _]
          tunnel: [_ enum16{"Idle", "Initialize", "Exit"}."Exit" enum16{"Idle", "Initialize", "Exit"}."Exit" _ _ _ _ _ _ _ _ _ _ _ _ _ _ _ _ _ _ _ _ _] -> w1180
          tunnel: w1179 -> [w1182 w1191 _ _ _ _ _ _ _ _ _ _ _ _ _ _ _ _ _ _ _ _ _ _]
          tunnel: w1177 -> [w1185 _ w1200 w1202 w1211 w1219 w1232 w1247 w1259 w1271 w1273 w1287 w1294 w1301 w1308 w1324 w1356 w1379 w1408 w1437 w1467 w1501 w1534 w1564]
          tunnel: [w1183 w1190 w1200 w1201 w1207 w1218 w1231 w1246 w1258 w1270 w1274 w1288 w1295 w1302 w1309 w1325 w1357 w1380 w1409 w1438 w1468 w1502 w1535 w1565] -> w1178
          tunnel: [-1 _ _ _ _ _ _ _ _ _ _ _ _ _ _ _ _ _ _ _ _ _ _ _] -> w1176
          tunnel: w1172 -> [w1181 w1189 w1198 w1204 w1212 w1220 w1233 w1248 w1260 w1272 w1280 w1289 w1296 w1303 w1310 w1330 w1362 w1390 w1419 w1448 w1478 w1512 w1545 w1566]
          tunnel: [w1181 w1189 w1198 w1204 w1212 w1220 w1233 w1248 w1260 w1272 w1280 w1289 w1296 w1303 w1310 w1330 w1362 w1390 w1419 w1448 w1478 w1512 w1545 w1566] -> w1171
          event Timeout {
            n518 = event-data() -> ()  [unwired: 1 in, 3 out]
            n519 = call-poly <userlib>:"CSM - Filter JKISM String Queue.vi"("States In"=w1185) -> ("States Out"=w1184:string)  [unwired: 14 in]
            n520 = call <userlib>:"CSM - Forward UI Operations to CSM.vi"("Name (\"\" to Use UUID)"=w1182, "State(s) In (\"\")"=w1184) -> ("States Out"=w1183:string)  [unwired: 8 in, 1 out]
          }
          event Panel Close? {
            # "#CSM \nIf you use this as the topmost VI\nDo not set it to FALSE"
            n521 = event-data() -> ()  [unwired: 1 in, 1 out]
            n522 = Two Button Dialog(message="确定关闭程序？" ("消息")) -> (T button?=w1187:bool)  [unwired: 2 in]
            n523 = case shown="假" w1187 {
              tunnel: w1191 -> [w1194 w1196]
              tunnel: [w1194 w1195] -> w1190
              frame False {
              }
              frame True {
                n524 = call <userlib>:"CSM - Forward UI Operations to CSM.vi"("Name (\"\" to Use UUID)"=w1196, "State(s) In (\"\")"="Macro: Exit" ("State")) -> ("States Out"=w1195:string)  [unwired: 8 in, 1 out]
              }
            }
            n525 = event-data("Discard?"=TRUE) -> ()  [unwired: 1 in, 1 out]
          }
          event User Event {
            n526 = event-data() -> ()  [unwired: 1 in, 1 out]
          }
          event "停止": Value Change {
            n527 = event-data() -> ()  [unwired: 1 in, 1 out]
            n528 = call <vilib>:"Add State(s) to Queue__JKI_lib_State_Machine.vi"("State(s) in Front (\"\")"="Macro: Exit" ("State(s) in Front (\"\")"), "State(s) in (\"\")"=w1202) -> ("States Out"=w1201:string)  [unwired: 13 in]
          }
          event "打开串口": Value Change {
            n529 = event-data() -> ()  [unwired: 1 in, 1 out]
            n530 = call-poly <userlib>:"Add State(s) to Queue By BOOL++.vi"("FALSE (\"\")"="Macro: Stop" ("State(s) in Front (\"\")"), "TRUE (\"\")"="Macro: Start" ("State(s) in Front (\"\")"), "High Priority? (F)"=TRUE, "Condition"="打开串口", "State Queue (\"\")"=w1211) -> ("Remaining States"=w1207:string)  [unwired: 6 in]
            n531 = local write "温控-错误输出"(errorcluster {"status"=FALSE, "code"=0, "source"=""} ("错误常量")) -> ()
          }
          event "温控开关 1": Value Change {
            n532 = event-data() -> ("OldVal"=w1214:bool, "NewVal"=w1215:bool)  [unwired: 1 in]
            n533 = Not Equal?(x=w1214, y=w1215) -> (x != y?=w1213:bool)
            n534 = case shown="真" w1213 {
              tunnel: ["" ("State with Arguments") w1223] -> w1217
              tunnel: "温控开关 1" -> [_ w1222]
              frame False {
              }
              frame True {
                n535 = call "Convert Data To API String Arguments.vim"("Data"=w1222) -> ("API String"=w1225:string)  [unwired: 7 in, 1 out]
                n536 = call <vilib>:"Build State String with Arguments__JKI_lib_State_Machine.vi"("Arguments (\"\")"=w1225, "State"="Action: Power Output 1" ("State(s) in Front (\"\")")) -> ("State with Arguments"=w1223:string)  [unwired: 4 in]
              }
            }
            n537 = call <vilib>:"Add State(s) to Queue__JKI_lib_State_Machine.vi"("State(s) in Front (\"\")"=w1217, "State(s) in (\"\")"=w1219) -> ("States Out"=w1218:string)  [unwired: 13 in]
          }
          event "温控开关 2": Value Change {
            n538 = event-data() -> ("OldVal"=w1227:bool, "NewVal"=w1228:bool)  [unwired: 1 in]
            n539 = Not Equal?(x=w1227, y=w1228) -> (x != y?=w1226:bool)
            n540 = case shown="假" w1226 {
              tunnel: ["" ("State with Arguments") w1236] -> w1230
              tunnel: "温控开关 2" -> [_ w1235]
              frame False {
              }
              frame True {
                n541 = call "Convert Data To API String Arguments.vim"("Data"=w1235) -> ("API String"=w1238:string)  [unwired: 7 in, 1 out]
                n542 = call <vilib>:"Build State String with Arguments__JKI_lib_State_Machine.vi"("Arguments (\"\")"=w1238, "State"="Action: Power Output 2" ("State(s) in Front (\"\")")) -> ("State with Arguments"=w1236:string)  [unwired: 4 in]
              }
            }
            n543 = call <vilib>:"Add State(s) to Queue__JKI_lib_State_Machine.vi"("State(s) in Front (\"\")"=w1230, "State(s) in (\"\")"=w1232) -> ("States Out"=w1231:string)  [unwired: 13 in]
          }
          event "温控开关 总": Value Change {
            n544 = event-data() -> ()  [unwired: 1 in, 1 out]
            n545 = call "Convert Data To API String Arguments.vim"("Data"="温控开关 总") -> ("API String"=w1243:string)  [unwired: 7 in, 1 out]
            n546 = call <vilib>:"Build State String with Arguments__JKI_lib_State_Machine.vi"("Arguments (\"\")"=w1243, "State"="Action: Power Output 1" ("State(s) in Front (\"\")")) -> ("State with Arguments"=w1241:string)  [unwired: 4 in]
            n547 = call <vilib>:"Build State String with Arguments__JKI_lib_State_Machine.vi"("Arguments (\"\")"=w1243, "State"="Action: Power Output 2" ("State(s) in Front (\"\")")) -> ("State with Arguments"=w1240:string)  [unwired: 4 in]
            n548 = call <vilib>:"Add State(s) to Queue__JKI_lib_State_Machine.vi"("State(s) in Front (\"\")"=w1241, "State(s) in (\"\")"=w1240) -> ("States Out"=w1239:string)  [unwired: 13 in]
            n549 = call <vilib>:"Add State(s) to Queue__JKI_lib_State_Machine.vi"("State(s) in Front (\"\")"=w1239, "State(s) in (\"\")"=w1247) -> ("States Out"=w1246:string)  [unwired: 13 in]
          }
          event "温控温度 1": Value Change {
            n550 = event-data() -> ("OldVal"=w1255:dbl, "NewVal"=w1254:dbl)  [unwired: 1 in, 1 out]
            n551 = Not Equal?(x=w1255, y=w1254) -> (x != y?=w1252:bool)
            n552 = call "Convert Data To API String Arguments.vim"("Data"="温控温度 1") -> ("API String"=w1257:string)  [unwired: 7 in, 1 out]
            n553 = call <vilib>:"Build State String with Arguments__JKI_lib_State_Machine.vi"("Arguments (\"\")"=w1257, "State"="Action: Change Temp 1" ("State(s) in Front (\"\")")) -> ("State with Arguments"=w1253:string)  [unwired: 4 in]
            n554 = Select(t=w1253, s=w1252, f="") -> (s? t:f=w1250:string)
            n555 = call <vilib>:"Add State(s) to Queue__JKI_lib_State_Machine.vi"("State(s) in Front (\"\")"=w1250, "State(s) in (\"\")"=w1259) -> ("States Out"=w1258:string)  [unwired: 13 in]
          }
          event "温控温度 2": Value Change {
            n556 = event-data() -> ("OldVal"=w1265:dbl, "NewVal"=w1266:dbl)  [unwired: 1 in, 1 out]
            n557 = Not Equal?(x=w1265, y=w1266) -> (x != y?=w1264:bool)
            n558 = call "Convert Data To API String Arguments.vim"("Data"="温控温度 2") -> ("API String"=w1269:string)  [unwired: 7 in, 1 out]
            n559 = call <vilib>:"Build State String with Arguments__JKI_lib_State_Machine.vi"("Arguments (\"\")"=w1269, "State"="Action: Change Temp 2" ("State(s) in Front (\"\")")) -> ("State with Arguments"=w1263:string)  [unwired: 4 in]
            n560 = Select(t=w1263, s=w1264, f="") -> (s? t:f=w1262:string)
            n561 = call <vilib>:"Add State(s) to Queue__JKI_lib_State_Machine.vi"("State(s) in Front (\"\")"=w1262, "State(s) in (\"\")"=w1271) -> ("States Out"=w1270:string)  [unwired: 13 in]
          }
          event "温度": Value Change {
            n562 = event-data() -> ()  [unwired: 1 in, 1 out]
            n563 = Select(t="温控温度 A", s="温度", f="温控温度 B") -> (s? t:f=w1275:dbl)
            n564 = case shown="真" "通道" {
              tunnel: w1275 -> [w1281 w1282]
              frame False {
                n565 = property on="温控温度 2" class="DigNum (严格)"("Val(Sgnl)"=w1281) -> ()  [unwired: 2 in, 2 out]
              }
              frame True {
                n566 = property on="温控温度 1" class="DigNum (严格)"("Val(Sgnl)"=w1282) -> ()  [unwired: 2 in, 2 out]
              }
            }
            n567 = call <vilib>:"Add State(s) to Queue__JKI_lib_State_Machine.vi"("State(s) in (\"\")"=w1273) -> ("States Out"=w1274:string)  [unwired: 14 in]
          }
          event "电源切换 1": Value Change {
            n568 = event-data() -> ()  [unwired: 1 in, 1 out]
            n569 = call "Convert Data To API String Arguments.vim"("Data"="电源切换 1") -> ("API String"=w1286:string)  [unwired: 7 in, 1 out]
            n570 = call <vilib>:"Build State String with Arguments__JKI_lib_State_Machine.vi"("Arguments (\"\")"=w1286, "State"="Action: Power Switch 1") -> ("State with Arguments"=w1284:string)  [unwired: 4 in]
            n571 = call <vilib>:"Add State(s) to Queue__JKI_lib_State_Machine.vi"("State(s) in Front (\"\")"=w1284, "State(s) in (\"\")"=w1287) -> ("States Out"=w1288:string)  [unwired: 13 in]
          }
          event "电源切换 2": Value Change {
            n572 = event-data() -> ()  [unwired: 1 in, 1 out]
            n573 = call "Convert Data To API String Arguments.vim"("Data"="电源切换 2") -> ("API String"=w1293:string)  [unwired: 7 in, 1 out]
            n574 = call <vilib>:"Build State String with Arguments__JKI_lib_State_Machine.vi"("Arguments (\"\")"=w1293, "State"="Action: Power Switch 2") -> ("State with Arguments"=w1291:string)  [unwired: 4 in]
            n575 = call <vilib>:"Add State(s) to Queue__JKI_lib_State_Machine.vi"("State(s) in Front (\"\")"=w1291, "State(s) in (\"\")"=w1294) -> ("States Out"=w1295:string)  [unwired: 13 in]
          }
          event "Fast Mode": Value Change {
            n576 = event-data() -> ()  [unwired: 1 in, 1 out]
            n577 = call "Convert Data To API String Arguments.vim"("Data"="Fast Mode") -> ("API String"=w1298:string)  [unwired: 7 in, 1 out]
            n578 = call <vilib>:"Build State String with Arguments__JKI_lib_State_Machine.vi"("Arguments (\"\")"=w1298, "State"="Acq: Fast Mode") -> ("State with Arguments"=w1299:string)  [unwired: 4 in]
            n579 = call <vilib>:"Add State(s) to Queue__JKI_lib_State_Machine.vi"("State(s) in Front (\"\")"=w1299, "State(s) in (\"\")"=w1301) -> ("States Out"=w1302:string)  [unwired: 13 in]
          }
          event "采集间隔": Value Change {
            n580 = event-data() -> ()  [unwired: 1 in, 1 out]
            n581 = call "Convert Data To API String Arguments.vim"("Data"="采集间隔") -> ("API String"=w1305:string)  [unwired: 7 in, 1 out]
            n582 = call <vilib>:"Build State String with Arguments__JKI_lib_State_Machine.vi"("Arguments (\"\")"=w1305, "State"="Acq: Sample Interval") -> ("State with Arguments"=w1306:string)  [unwired: 4 in]
            n583 = call <vilib>:"Add State(s) to Queue__JKI_lib_State_Machine.vi"("State(s) in Front (\"\")"=w1306, "State(s) in (\"\")"=w1308) -> ("States Out"=w1309:string)  [unwired: 13 in]
          }
          event "输出设置 1": Value Change {
            n584 = event-data() -> ("OldVal"=w1327:T4, "NewVal"=w1326:T4)  [unwired: 1 in, 1 out]
            n585 = Not Equal?(x=w1327, y=w1326) -> (x != y?=w1328:cluster{"输出模式":bool, "最大输出电压":bool})
            n586 = Cluster To Array(cluster=w1328) -> (array=w1329:bool[])
            n587 = Boolean Array To Number(Boolean array=w1329) -> (number=w1319:u32)
            n588 = Number To Decimal String(number=w1319) -> (decimal integer string=w1321:string)  [unwired: 1 in]
            n589 = case shown="1" w1319 {
              tunnel: "输出设置 1" -> [_ w1340 w1342]
              tunnel: [_ w1339 w1341] -> w1320
              frame 0, Default {
              }
              frame 1 {
                n590 = Unbundle By Name(w1340) -> ("输出模式"=w1339:enum16{"致冷模式", "加热模式", "双向模式"})
              }
              frame 2 {
                n591 = Unbundle By Name(w1342) -> ("最大输出电压"=w1341:dbl)
              }
            }
            n592 = local read "温控开关 1"() -> (w1313:bool)
            n593 = Number To Fractional String(number=w1320) -> (F-format string=w1318:string)  [unwired: 3 in]
            n594 = Concatenate Strings(w1321, "/" ("字符串"), w1318) -> (w1317:string)
            n595 = case shown="真" w1313 {
              tunnel: [w1331 w1333] -> w1312
              tunnel: [w1331 w1332] -> w1311
              frame False {
                w1331 = "" ("State with Arguments")
              }
              frame True {
                w1334 = "Action: Power Output 1"
                n596 = call "Convert Data To API String Arguments.vim"("Data"=TRUE) -> ("API String"=w1335:string)  [unwired: 7 in, 1 out]
                n597 = call "Convert Data To API String Arguments.vim"("Data"=FALSE) -> ("API String"=w1336:string)  [unwired: 7 in, 1 out]
                n598 = call <vilib>:"Build State String with Arguments__JKI_lib_State_Machine.vi"("Arguments (\"\")"=w1336, "State"=w1334) -> ("State with Arguments"=w1333:string)  [unwired: 4 in]
                n599 = call <vilib>:"Build State String with Arguments__JKI_lib_State_Machine.vi"("Arguments (\"\")"=w1335, "State"=w1334) -> ("State with Arguments"=w1332:string)  [unwired: 4 in]
              }
            }
            n600 = call <vilib>:"Build State String with Arguments__JKI_lib_State_Machine.vi"("Arguments (\"\")"=w1317, "State"="Action: Output Set 1") -> ("State with Arguments"=w1314:string)  [unwired: 4 in]
            n601 = call <vilib>:"Add State(s) to Queue__JKI_lib_State_Machine.vi"("State(s) in Front (\"\")"=w1312, "State(s) in (\"\")"=w1314, "State(s) at Back (\"\")"=w1311) -> ("States Out"=w1315:string)  [unwired: 12 in]
            n602 = call <vilib>:"Add State(s) to Queue__JKI_lib_State_Machine.vi"("State(s) in Front (\"\")"=w1315, "State(s) in (\"\")"=w1324) -> ("States Out"=w1325:string)  [unwired: 13 in]
          }
          event "输出设置 2": Value Change {
            n603 = event-data() -> ("OldVal"=w1359:T4, "NewVal"=w1358:T4)  [unwired: 1 in, 1 out]
            n604 = Not Equal?(x=w1359, y=w1358) -> (x != y?=w1360:cluster{"输出模式":bool, "最大输出电压":bool})
            n605 = Cluster To Array(cluster=w1360) -> (array=w1361:bool[])
            n606 = Boolean Array To Number(Boolean array=w1361) -> (number=w1351:u32)
            n607 = Number To Decimal String(number=w1351) -> (decimal integer string=w1353:string)  [unwired: 1 in]
            n608 = case shown="1" w1351 {
              tunnel: "输出设置 2" -> [_ w1372 w1374]
              tunnel: [_ w1371 w1373] -> w1352
              frame 0, Default {
              }
              frame 1 {
                n609 = Unbundle By Name(w1372) -> ("输出模式"=w1371:enum16{"致冷模式", "加热模式", "双向模式"})
              }
              frame 2 {
                n610 = Unbundle By Name(w1374) -> ("最大输出电压"=w1373:dbl)
              }
            }
            n611 = Number To Fractional String(number=w1352) -> (F-format string=w1350:string)  [unwired: 3 in]
            n612 = local read "温控开关 2"() -> (w1343:bool)
            n613 = Concatenate Strings(w1353, "/" ("字符串"), w1350) -> (w1349:string)
            n614 = call <vilib>:"Build State String with Arguments__JKI_lib_State_Machine.vi"("Arguments (\"\")"=w1349, "State"="Action: Output Set 2") -> ("State with Arguments"=w1345:string)  [unwired: 4 in]
            n615 = case shown="真" w1343 {
              tunnel: [w1363 w1365] -> w1347
              tunnel: [w1363 w1364] -> w1346
              frame False {
                w1363 = "" ("State with Arguments")
              }
              frame True {
                w1366 = "Action: Power Output 2"
                n616 = call "Convert Data To API String Arguments.vim"("Data"=TRUE) -> ("API String"=w1367:string)  [unwired: 7 in, 1 out]
                n617 = call "Convert Data To API String Arguments.vim"("Data"=FALSE) -> ("API String"=w1368:string)  [unwired: 7 in, 1 out]
                n618 = call <vilib>:"Build State String with Arguments__JKI_lib_State_Machine.vi"("Arguments (\"\")"=w1368, "State"=w1366) -> ("State with Arguments"=w1365:string)  [unwired: 4 in]
                n619 = call <vilib>:"Build State String with Arguments__JKI_lib_State_Machine.vi"("Arguments (\"\")"=w1367, "State"=w1366) -> ("State with Arguments"=w1364:string)  [unwired: 4 in]
              }
            }
            n620 = call <vilib>:"Add State(s) to Queue__JKI_lib_State_Machine.vi"("State(s) in Front (\"\")"=w1347, "State(s) in (\"\")"=w1345, "State(s) at Back (\"\")"=w1346) -> ("States Out"=w1344:string)  [unwired: 12 in]
            n621 = call <vilib>:"Add State(s) to Queue__JKI_lib_State_Machine.vi"("State(s) in Front (\"\")"=w1344, "State(s) in (\"\")"=w1356) -> ("States Out"=w1357:string)  [unwired: 13 in]
          }
          event "PID 1": Value Change {
            n622 = event-data() -> ("OldVal"=w1382:T5, "NewVal"=w1381:T5)  [unwired: 1 in, 4 out]
            n623 = Not Equal?(x=w1382, y=w1381) -> (x != y?=w1389:T23)
            n624 = Cluster To Array(cluster=w1389) -> (array=w1388:bool[])
            n625 = Boolean Array To Number(Boolean array=w1388) -> (number=w1387:u32)
            n626 = case shown="1" w1387 {
              tunnel: "PID 1" -> [_ w1393 w1395 w1397 w1399 w1401 w1403]
              tunnel: [0.0 ("PID控制间隔") w1392 w1394 w1396 w1398 w1400 w1402] -> w1386
              frame 0, Default {
              }
              frame 1 {
                n627 = Unbundle By Name(w1393) -> ("PID类型"=w1392:enum16{"P", "PI", "PID"})
              }
              frame 2 {
                n628 = Unbundle By Name(w1395) -> ("P"=w1394:dbl)
              }
              frame 4 {
                n629 = Unbundle By Name(w1397) -> ("I"=w1396:dbl)
              }
              frame 8 {
                n630 = Unbundle By Name(w1399) -> ("D"=w1398:dbl)
              }
              frame 16 {
                n631 = Unbundle By Name(w1401) -> ("PID控制间隔"=w1400:dbl)
              }
              frame 32 {
                n632 = Unbundle By Name(w1403) -> ("PID计算方法"=w1402:enum16{"位置式", "增量式", "最大正向输出", "最大负向输出"})
              }
            }
            n633 = Number To Decimal String(number=w1387) -> (decimal integer string=w1385:string)  [unwired: 1 in]
            n634 = Number To Fractional String(number=w1386) -> (F-format string=w1384:string)  [unwired: 3 in]
            n635 = Concatenate Strings(w1385, "/" ("字符串"), w1384) -> (w1377:string)
            n636 = call <vilib>:"Build State String with Arguments__JKI_lib_State_Machine.vi"("Arguments (\"\")"=w1377, "State"="Action: PID Set 1") -> ("State with Arguments"=w1376:string)  [unwired: 4 in]
            n637 = call <vilib>:"Add State(s) to Queue__JKI_lib_State_Machine.vi"("State(s) in Front (\"\")"=w1376, "State(s) in (\"\")"=w1379) -> ("States Out"=w1380:string)  [unwired: 13 in]
          }
          event "PID 2": Value Change {
            n638 = event-data() -> ("OldVal"=w1411:T5, "NewVal"=w1410:T5)  [unwired: 1 in, 4 out]
            n639 = Not Equal?(x=w1411, y=w1410) -> (x != y?=w1418:T23)
            n640 = Cluster To Array(cluster=w1418) -> (array=w1417:bool[])
            n641 = Boolean Array To Number(Boolean array=w1417) -> (number=w1416:u32)
            n642 = case shown="1" w1416 {
              tunnel: "PID 2" -> [_ w1422 w1424 w1426 w1428 w1430 w1432]
              tunnel: [0.0 ("PID控制间隔") w1421 w1423 w1425 w1427 w1429 w1431] -> w1415
              frame 0, Default {
              }
              frame 1 {
                n643 = Unbundle By Name(w1422) -> ("PID类型"=w1421:enum16{"P", "PI", "PID"})
              }
              frame 2 {
                n644 = Unbundle By Name(w1424) -> ("P"=w1423:dbl)
              }
              frame 4 {
                n645 = Unbundle By Name(w1426) -> ("I"=w1425:dbl)
              }
              frame 8 {
                n646 = Unbundle By Name(w1428) -> ("D"=w1427:dbl)
              }
              frame 16 {
                n647 = Unbundle By Name(w1430) -> ("PID控制间隔"=w1429:dbl)
              }
              frame 32 {
                n648 = Unbundle By Name(w1432) -> ("PID计算方法"=w1431:enum16{"位置式", "增量式", "最大正向输出", "最大负向输出"})
              }
            }
            n649 = Number To Decimal String(number=w1416) -> (decimal integer string=w1414:string)  [unwired: 1 in]
            n650 = Number To Fractional String(number=w1415) -> (F-format string=w1413:string)  [unwired: 3 in]
            n651 = Concatenate Strings(w1414, "/" ("字符串"), w1413) -> (w1406:string)
            n652 = call <vilib>:"Build State String with Arguments__JKI_lib_State_Machine.vi"("Arguments (\"\")"=w1406, "State"="Action: PID Set 2") -> ("State with Arguments"=w1405:string)  [unwired: 4 in]
            n653 = call <vilib>:"Add State(s) to Queue__JKI_lib_State_Machine.vi"("State(s) in Front (\"\")"=w1405, "State(s) in (\"\")"=w1408) -> ("States Out"=w1409:string)  [unwired: 13 in]
          }
          event "过温 1": Value Change {
            n654 = event-data() -> ("OldVal"=w1440:T6, "NewVal"=w1439:T6)  [unwired: 1 in, 4 out]
            n655 = Not Equal?(x=w1440, y=w1439) -> (x != y?=w1447:T24)
            n656 = Cluster To Array(cluster=w1447) -> (array=w1446:bool[])
            n657 = Boolean Array To Number(Boolean array=w1446) -> (number=w1445:u32)
            n658 = case shown="0, 默认" w1445 {
              tunnel: "过温 1" -> [_ w1452 w1454 w1456 w1458 w1460 w1462]
              tunnel: [0.0 ("温度限速") w1450 w1453 w1455 w1457 w1459 w1461] -> w1444
              frame 0, Default {
              }
              frame 1 {
                n659 = Unbundle By Name(w1452) -> ("过温保护开关"=w1451:bool)
                n660 = Boolean To (0,1)(Boolean=w1451) -> (0, 1=w1450:i16)
              }
              frame 2 {
                n661 = Unbundle By Name(w1454) -> ("过温保护低阈值"=w1453:dbl)
              }
              frame 4 {
                n662 = Unbundle By Name(w1456) -> ("过温保护高阈值"=w1455:dbl)
              }
              frame 8 {
                n663 = Unbundle By Name(w1458) -> ("最低设定温度"=w1457:dbl)
              }
              frame 16 {
                n664 = Unbundle By Name(w1460) -> ("最高设定温度"=w1459:dbl)
              }
              frame 32 {
                n665 = Unbundle By Name(w1462) -> ("温度限速"=w1461:dbl)
              }
            }
            n666 = Number To Decimal String(number=w1445) -> (decimal integer string=w1443:string)  [unwired: 1 in]
            n667 = Number To Fractional String(number=w1444) -> (F-format string=w1442:string)  [unwired: 3 in]
            n668 = Concatenate Strings(w1443, "/" ("字符串"), w1442) -> (w1435:string)
            n669 = call <vilib>:"Build State String with Arguments__JKI_lib_State_Machine.vi"("Arguments (\"\")"=w1435, "State"="Action: OTP Set 1") -> ("State with Arguments"=w1434:string)  [unwired: 4 in]
            n670 = call <vilib>:"Add State(s) to Queue__JKI_lib_State_Machine.vi"("State(s) in Front (\"\")"=w1434, "State(s) in (\"\")"=w1437) -> ("States Out"=w1438:string)  [unwired: 13 in]
          }
          event "过温 2": Value Change {
            n671 = event-data() -> ("OldVal"=w1470:T6, "NewVal"=w1469:T6)  [unwired: 1 in, 4 out]
            n672 = Not Equal?(x=w1470, y=w1469) -> (x != y?=w1477:T24)
            n673 = Cluster To Array(cluster=w1477) -> (array=w1476:bool[])
            n674 = Boolean Array To Number(Boolean array=w1476) -> (number=w1475:u32)
            n675 = case shown="0, 默认" w1475 {
              tunnel: "过温 2" -> [_ w1482 w1484 w1486 w1488 w1490 w1492]
              tunnel: [0.0 ("温度限速") w1480 w1483 w1485 w1487 w1489 w1491] -> w1474
              frame 0, Default {
              }
              frame 1 {
                n676 = Unbundle By Name(w1482) -> ("过温保护开关"=w1481:bool)
                n677 = Boolean To (0,1)(Boolean=w1481) -> (0, 1=w1480:i16)
              }
              frame 2 {
                n678 = Unbundle By Name(w1484) -> ("过温保护低阈值"=w1483:dbl)
              }
              frame 4 {
                n679 = Unbundle By Name(w1486) -> ("过温保护高阈值"=w1485:dbl)
              }
              frame 8 {
                n680 = Unbundle By Name(w1488) -> ("最低设定温度"=w1487:dbl)
              }
              frame 16 {
                n681 = Unbundle By Name(w1490) -> ("最高设定温度"=w1489:dbl)
              }
              frame 32 {
                n682 = Unbundle By Name(w1492) -> ("温度限速"=w1491:dbl)
              }
            }
            n683 = Number To Decimal String(number=w1475) -> (decimal integer string=w1473:string)  [unwired: 1 in]
            n684 = Number To Fractional String(number=w1474) -> (F-format string=w1472:string)  [unwired: 3 in]
            n685 = Concatenate Strings(w1473, "/" ("字符串"), w1472) -> (w1465:string)
            n686 = call <vilib>:"Build State String with Arguments__JKI_lib_State_Machine.vi"("Arguments (\"\")"=w1465, "State"="Action: OTP Set 2") -> ("State with Arguments"=w1464:string)  [unwired: 4 in]
            n687 = call <vilib>:"Add State(s) to Queue__JKI_lib_State_Machine.vi"("State(s) in Front (\"\")"=w1464, "State(s) in (\"\")"=w1467) -> ("States Out"=w1468:string)  [unwired: 13 in]
          }
          event "过压/过流 1": Value Change {
            n688 = event-data() -> ("OldVal"=w1504:cluster{"过压保护阈值":dbl, "过流保护阈值":dbl}, "NewVal"=w1503:cluster{"过压保护阈值":dbl, "过流保护阈值":dbl})  [unwired: 1 in]
            n689 = Not Equal?(x=w1504, y=w1503) -> (x != y?=w1511:cluster{"过压保护阈值":bool, "过流保护阈值":bool})
            n690 = Cluster To Array(cluster=w1511) -> (array=w1510:bool[])
            n691 = Boolean Array To Number(Boolean array=w1510) -> (number=w1509:u32)
            n692 = case shown="1" w1509 {
              tunnel: "过压/过流 1" -> [_ w1523 w1525]
              tunnel: [0.0 ("过流保护阈值") w1522 w1524] -> w1508
              frame 0, Default {
              }
              frame 1 {
                n693 = Unbundle By Name(w1523) -> ("过压保护阈值"=w1522:dbl)
              }
              frame 2 {
                n694 = Unbundle By Name(w1525) -> ("过流保护阈值"=w1524:dbl)
              }
            }
            n695 = Number To Decimal String(number=w1509) -> (decimal integer string=w1507:string)  [unwired: 1 in]
            n696 = local read "温控开关 1"() -> (w1493:bool)
            n697 = Number To Fractional String(number=w1508) -> (F-format string=w1506:string)  [unwired: 3 in]
            n698 = Concatenate Strings(w1507, "/" ("字符串"), w1506) -> (w1499:string)
            n699 = case shown="真" w1493 {
              tunnel: [w1513 w1515] -> w1497
              tunnel: [w1513 w1514] -> w1496
              frame False {
                w1513 = "" ("State with Arguments")
              }
              frame True {
                w1516 = "Action: Power Output 1"
                n700 = call "Convert Data To API String Arguments.vim"("Data"=TRUE) -> ("API String"=w1517:string)  [unwired: 7 in, 1 out]
                n701 = call "Convert Data To API String Arguments.vim"("Data"=FALSE) -> ("API String"=w1518:string)  [unwired: 7 in, 1 out]
                n702 = call <vilib>:"Build State String with Arguments__JKI_lib_State_Machine.vi"("Arguments (\"\")"=w1518, "State"=w1516) -> ("State with Arguments"=w1515:string)  [unwired: 4 in]
                n703 = call <vilib>:"Build State String with Arguments__JKI_lib_State_Machine.vi"("Arguments (\"\")"=w1517, "State"=w1516) -> ("State with Arguments"=w1514:string)  [unwired: 4 in]
              }
            }
            n704 = call <vilib>:"Build State String with Arguments__JKI_lib_State_Machine.vi"("Arguments (\"\")"=w1499, "State"="Action: OVP Set 1") -> ("State with Arguments"=w1495:string)  [unwired: 4 in]
            n705 = call <vilib>:"Add State(s) to Queue__JKI_lib_State_Machine.vi"("State(s) in Front (\"\")"=w1497, "State(s) in (\"\")"=w1495, "State(s) at Back (\"\")"=w1496) -> ("States Out"=w1494:string)  [unwired: 12 in]
            n706 = call <vilib>:"Add State(s) to Queue__JKI_lib_State_Machine.vi"("State(s) in Front (\"\")"=w1494, "State(s) in (\"\")"=w1501) -> ("States Out"=w1502:string)  [unwired: 13 in]
          }
          event "过压/过流 2": Value Change {
            n707 = event-data() -> ("OldVal"=w1537:cluster{"过压保护阈值":dbl, "过流保护阈值":dbl}, "NewVal"=w1536:cluster{"过压保护阈值":dbl, "过流保护阈值":dbl})  [unwired: 1 in]
            n708 = Not Equal?(x=w1537, y=w1536) -> (x != y?=w1544:cluster{"过压保护阈值":bool, "过流保护阈值":bool})
            n709 = Cluster To Array(cluster=w1544) -> (array=w1543:bool[])
            n710 = Boolean Array To Number(Boolean array=w1543) -> (number=w1542:u32)
            n711 = case shown="2" w1542 {
              tunnel: "过压/过流 2" -> [_ w1556 w1558]
              tunnel: [0.0 ("过流保护阈值") w1555 w1557] -> w1541
              frame 0, Default {
              }
              frame 1 {
                n712 = Unbundle By Name(w1556) -> ("过压保护阈值"=w1555:dbl)
              }
              frame 2 {
                n713 = Unbundle By Name(w1558) -> ("过流保护阈值"=w1557:dbl)
              }
            }
            n714 = Number To Decimal String(number=w1542) -> (decimal integer string=w1540:string)  [unwired: 1 in]
            n715 = Number To Fractional String(number=w1541) -> (F-format string=w1539:string)  [unwired: 3 in]
            n716 = local read "温控开关 2"() -> (w1526:bool)
            n717 = Concatenate Strings(w1540, "/" ("字符串"), w1539) -> (w1532:string)
            n718 = call <vilib>:"Build State String with Arguments__JKI_lib_State_Machine.vi"("Arguments (\"\")"=w1532, "State"="Action: OVP Set 2") -> ("State with Arguments"=w1528:string)  [unwired: 4 in]
            n719 = case shown="真" w1526 {
              tunnel: [w1546 w1548] -> w1530
              tunnel: [w1546 w1547] -> w1529
              frame False {
                w1546 = "" ("State with Arguments")
              }
              frame True {
                w1549 = "Action: Power Output 2"
                n720 = call "Convert Data To API String Arguments.vim"("Data"=TRUE) -> ("API String"=w1550:string)  [unwired: 7 in, 1 out]
                n721 = call "Convert Data To API String Arguments.vim"("Data"=FALSE) -> ("API String"=w1551:string)  [unwired: 7 in, 1 out]
                n722 = call <vilib>:"Build State String with Arguments__JKI_lib_State_Machine.vi"("Arguments (\"\")"=w1551, "State"=w1549) -> ("State with Arguments"=w1548:string)  [unwired: 4 in]
                n723 = call <vilib>:"Build State String with Arguments__JKI_lib_State_Machine.vi"("Arguments (\"\")"=w1550, "State"=w1549) -> ("State with Arguments"=w1547:string)  [unwired: 4 in]
              }
            }
            n724 = call <vilib>:"Add State(s) to Queue__JKI_lib_State_Machine.vi"("State(s) in Front (\"\")"=w1530, "State(s) in (\"\")"=w1528, "State(s) at Back (\"\")"=w1529) -> ("States Out"=w1527:string)  [unwired: 12 in]
            n725 = call <vilib>:"Add State(s) to Queue__JKI_lib_State_Machine.vi"("State(s) in Front (\"\")"=w1527, "State(s) in (\"\")"=w1534) -> ("States Out"=w1535:string)  [unwired: 13 in]
          }
          event "温控循环功能开启": Value Change {
            n726 = event-data() -> ("OldVal"=w1560:bool, "NewVal"=w1561:bool)  [unwired: 1 in, 4 out]
            n727 = Not Equal?(x=w1560, y=w1561) -> (x != y?=w1559:bool)
            n728 = case shown="真" w1559 {
              tunnel: ["" w1569] -> w1563
              tunnel: "温控循环功能开启" -> [_ w1568]
              frame False {
              }
              frame True {
                n729 = Select(t="Repeat: Enable", s=w1568, f="Repeat: Disable") -> (s? t:f=w1569:string)
              }
            }
            n730 = call <vilib>:"Add State(s) to Queue__JKI_lib_State_Machine.vi"("State(s) in Front (\"\")"=w1563, "State(s) in (\"\")"=w1564) -> ("States Out"=w1565:string)  [unwired: 13 in]
          }
        }
      }
      frame "Exit" {
        n731 = Unregister For Events(event registration refnum=w1574) -> (error out=w1573:errorcluster)  [unwired: 1 in]
        n732 = call <vilib>:"Clear Errors.vi"("error in (no error)"=w1573) -> ()  [unwired: 5 in, 2 out]
      }
    }
  }
  n733 = call <userlib>:"CSM - Sync Configuration Variables to File.vi"("All Temp Variable to Default Ini(F)"=TRUE, "error in (no error)"=w4) -> ()  [unwired: 7 in, 1 out]
